vi "ConvertTextBasedCodeToLabVIEW_CreateClasses.vi"(0 "Classes":T11[](array[typedef])=[{"ClassName"="Program", "AccessScope"=enum."public", "Modifiers"=[], "ClassDocumentation"="", "Methods"=[{"ReturnType"={"Name"="", "DataType"=enum."void", "ArrayDim"=0, "CtrlPath"=path "", "DataTypeString"="void", "AccessScope"=enum."public", "InitialData"=variant(string "")}, "MethodName"="Main", "AccessScope"=enum."public", "Modifiers"=[enum."static"], "MethodDocumentation"="", "MethodContent"="public static void Main(string[] args)\n        {\n            // Create a subject and the observable, inject the subject into the observable\n            Subject subject = new Subject();\n            SubjectObservable observable = new SubjectObservable(subject);\n\n            //Create two observers\n            SubjectObserver zeus = new SubjectObserver(observable, \"Zeus\");\n            SubjectObserver ares = new SubjectObserver(observable, \"Ares\");\n            \n            // Run a loop and trigger the observer\n            for (int i = 0; i < 5; i++)\n            {\n                Console.WriteLine(\"Counter: \" + subject.Counter);\n                observable.inspectSubject();\n\n            }\n\n            Console.ReadLine();\n        }", "MethodArguments"=[{"Name"="args", "DataType"=enum."STRING", "ArrayDim"=1, "CtrlPath"=path "", "DataTypeString"="string[]", "AccessScope"=enum."public", "InitialData"=variant(string "")}], "GetProperty"={"Active"=FALSE, "AccessScope"=enum."public", "Code"=""}, "SetProperty"={"Active"=FALSE, "AccessScope"=enum."public", "Code"=""}}], "ParentClasses"=[], "ClassType"=enum."Class", "Owner"="Test", "OwnerType"=enum."Package/NameSpace", "Generics"=[], "Attributes"=[{"Name"="MyUINT8", "DataType"=enum."UINT8", "ArrayDim"=0, "CtrlPath"=path "", "DataTypeString"="", "AccessScope"=enum."public", "InitialData"=variant}], "Enums"=[{"Name"="MyEnum", "AccessScope"=enum."public", "Modifiers"=[], "Items"=["A1", "A2"], "Documentation"="My Enum Doc"}], "Structs"=[{"Name"="MyStruct", "AccessScope"=enum."public", "Modifiers"=[], "Items"=[{"Name"="MyObject", "DataType"=enum."LabVIEW Class", "ArrayDim"=1, "CtrlPath"=path "", "DataTypeString"="Program", "AccessScope"=enum."public", "InitialData"=variant}, {"Name"="Sträng", "DataType"=enum."STRING", "ArrayDim"=0, "CtrlPath"=path "", "DataTypeString"="", "AccessScope"=enum."public", "InitialData"=variant}], "Documentation"="Struct Doc"}]}, {"ClassName"="Subject", "AccessScope"=enum."public", "Modifiers"=[], "ClassDocumentation"="Class Subject - It has a counter object that increases everytime you inspect it", "Methods"=[{"ReturnType"={"Name"="", "DataType"=enum."INT32", "ArrayDim"=0, "CtrlPath"=path "", "DataTypeString"="int", "AccessScope"=enum."public", "InitialData"=variant(string "")}, "MethodName"="Counter", "AccessScope"=enum."public", "Modifiers"=[], "MethodDocumentation"="", "MethodContent"="public int Counter\n        {\n            get\n            {\n                return ++_counter;\n            }\n        }", "MethodArguments"=[], "GetProperty"={"Active"=TRUE, "AccessScope"=enum."public", "Code"="return ++_counter;"}, "SetProperty"={"Active"=FALSE, "AccessScope"=enum."public", "Code"=""}}], "ParentClasses"=[], "ClassType"=enum."Class", "Owner"="Test", "OwnerType"=enum."Package/NameSpace", "Generics"=[], "Attributes"=[{"Name"="_counter", "DataType"=enum."INT32", "ArrayDim"=0, "CtrlPath"=path "", "DataTypeString"="int", "AccessScope"=enum."private", "InitialData"=variant(string "")}], "Enums"=[], "Structs"=[]}, {"ClassName"="SubjectObservable", "AccessScope"=enum."public", "Modifiers"=[], "ClassDocumentation"="Class Subject Observable - The observable object that observes the subject and notifies the observers", "Methods"=[{"ReturnType"={"Name"="", "DataType"=enum."LabVIEW Object", "ArrayDim"=0, "CtrlPath"=path "", "DataTypeString"="SubjectObservable", "AccessScope"=enum."public", "InitialData"=variant(string "")}, "MethodName"="SubjectObservable", "AccessScope"=enum."public", "Modifiers"=[], "MethodDocumentation"="Accept a subject instance which we shall observe", "MethodContent"="public SubjectObservable(Subject subject)\n        {\n            _subjectObservers = new List<IObserver<Subject>>();\n            _subject = subject;\n\n        }", "MethodArguments"=[{"Name"="subject", "DataType"=enum."LabVIEW Object", "ArrayDim"=0, "CtrlPath"=path "", "DataTypeString"="Subject", "AccessScope"=enum."public", "InitialData"=variant(string "")}], "GetProperty"={"Active"=FALSE, "AccessScope"=enum."public", "Code"=""}, "SetProperty"={"Active"=FALSE, "AccessScope"=enum."public", "Code"=""}}, {"ReturnType"={"Name"="", "DataType"=enum."Other", "ArrayDim"=0, "CtrlPath"=path "", "DataTypeString"="IDisposable", "AccessScope"=enum."public", "InitialData"=variant(string "")}, "MethodName"="Subscribe", "AccessScope"=enum."public", "Modifiers"=[], "MethodDocumentation"="This method allows the observers to attach themselves. It returns a disposer object to the observer\nwhich the observer can utilize to unsubscribe", "MethodContent"="public IDisposable Subscribe(IObserver<Subject> observer)\n        {\n            if (!_subjectObservers.Contains(observer))\n            {\n                _subjectObservers.Add(observer);\n            }\n\n            return new Disposer(_subjectObservers, observer);\n        }", "MethodArguments"=[{"Name"="observer", "DataType"=enum."Other", "ArrayDim"=0, "CtrlPath"=path "", "DataTypeString"="IObserver<Subject>", "AccessScope"=enum."public", "InitialData"=variant(string "")}], "GetProperty"={"Active"=FALSE, "AccessScope"=enum."public", "Code"=""}, "SetProperty"={"Active"=FALSE, "AccessScope"=enum."public", "Code"=""}}, {"ReturnType"={"Name"="", "DataType"=enum."void", "ArrayDim"=0, "CtrlPath"=path "", "DataTypeString"="void", "AccessScope"=enum."public", "InitialData"=variant(string "")}, "MethodName"="inspectSubject", "AccessScope"=enum."public", "Modifiers"=[enum."event"], "MethodDocumentation"="This method is used to inspect the subject over time. Usually used with a timer or an event", "MethodContent"="event\n        public void inspectSubject()\n        {\n            foreach (IObserver<Subject> observer in _subjectObservers)\n            {\n                observer.OnNext(_subject);\n            }\n        }", "MethodArguments"=[], "GetProperty"={"Active"=FALSE, "AccessScope"=enum."public", "Code"=""}, "SetProperty"={"Active"=FALSE, "AccessScope"=enum."public", "Code"=""}}], "ParentClasses"=[{"ClassName"="IObservable", "ClassType"=enum."Undefined"}], "ClassType"=enum."Class", "Owner"="Test", "OwnerType"=enum."Package/NameSpace", "Generics"=["Subject"], "Attributes"=[{"Name"="_subjectObservers", "DataType"=enum."Other", "ArrayDim"=1, "CtrlPath"=path "", "DataTypeString"="IObserver<Subject>", "AccessScope"=enum."private", "InitialData"=variant(string "")}, {"Name"="_subject", "DataType"=enum."LabVIEW Object", "ArrayDim"=0, "CtrlPath"=path "", "DataTypeString"="Subject", "AccessScope"=enum."private", "InitialData"=variant(string "")}], "Enums"=[], "Structs"=[]}, {"ClassName"="SubjectObserver", "AccessScope"=enum."public", "Modifiers"=[], "ClassDocumentation"="Class Subject Observer - The object that attaches itself to a observable and recieves notifications", "Methods"=[{"ReturnType"={"Name"="", "DataType"=enum."LabVIEW Object", "ArrayDim"=0, "CtrlPath"=path "", "DataTypeString"="SubjectObserver", "AccessScope"=enum."public", "InitialData"=variant(string "")}, "MethodName"="SubjectObserver", "AccessScope"=enum."public", "Modifiers"=[], "MethodDocumentation"="", "MethodContent"="public SubjectObserver(IObservable<Subject> provider, string instanceName)\n        {\n            if (provider != null)\n            {\n                _disposer = provider.Subscribe(this);\n                _instaceName = instanceName;\n            }\n        }", "MethodArguments"=[{"Name"="provider", "DataType"=enum."Other", "ArrayDim"=0, "CtrlPath"=path "", "DataTypeString"="IObservable<Subject>", "AccessScope"=enum."public", "InitialData"=variant(string "")}, {"Name"="instanceName", "DataType"=enum."STRING", "ArrayDim"=0, "CtrlPath"=path "", "DataTypeString"="string", "AccessScope"=enum."public", "InitialData"=variant(string "")}], "GetProperty"={"Active"=FALSE, "AccessScope"=enum."public", "Code"=""}, "SetProperty"={"Active"=FALSE, "AccessScope"=enum."public", "Code"=""}}, {"ReturnType"={"Name"="", "DataType"=enum."void", "ArrayDim"=0, "CtrlPath"=path "", "DataTypeString"="void", "AccessScope"=enum."public", "InitialData"=variant(string "")}, "MethodName"="OnNext", "AccessScope"=enum."public", "Modifiers"=[], "MethodDocumentation"="The observable invokes this method to pass the Subject object to the observer", "MethodContent"="public void OnNext(Subject value)\n        {\n            Console.WriteLine(\"[\" + _instaceName + \"] \" + value.Counter);\n        }", "MethodArguments"=[{"Name"="value", "DataType"=enum."LabVIEW Object", "ArrayDim"=0, "CtrlPath"=path "", "DataTypeString"="Subject", "AccessScope"=enum."public", "InitialData"=variant(string "")}], "GetProperty"={"Active"=FALSE, "AccessScope"=enum."public", "Code"=""}, "SetProperty"={"Active"=FALSE, "AccessScope"=enum."public", "Code"=""}}, {"ReturnType"={"Name"="", "DataType"=enum."void", "ArrayDim"=0, "CtrlPath"=path "", "DataTypeString"="void", "AccessScope"=enum."public", "InitialData"=variant(string "")}, "MethodName"="OnCompleted", "AccessScope"=enum."public", "Modifiers"=[], "MethodDocumentation"="Usually called when a transmission is complete. Not implemented.", "MethodContent"="public void OnCompleted()\n        {\n            throw new NotImplementedException();\n        }", "MethodArguments"=[], "GetProperty"={"Active"=FALSE, "AccessScope"=enum."public", "Code"=""}, "SetProperty"={"Active"=FALSE, "AccessScope"=enum."public", "Code"=""}}, {"ReturnType"={"Name"="", "DataType"=enum."void", "ArrayDim"=0, "CtrlPath"=path "", "DataTypeString"="void", "AccessScope"=enum."public", "InitialData"=variant(string "")}, "MethodName"="OnError", "AccessScope"=enum."public", "Modifiers"=[], "MethodDocumentation"="Usually called when there was an error. Didn't implement.", "MethodContent"="public void OnError(Exception error)\n        {\n            throw new NotImplementedException();\n        }", "MethodArguments"=[{"Name"="error", "DataType"=enum."Other", "ArrayDim"=0, "CtrlPath"=path "", "DataTypeString"="Exception", "AccessScope"=enum."public", "InitialData"=variant(string "")}], "GetProperty"={"Active"=FALSE, "AccessScope"=enum."public", "Code"=""}, "SetProperty"={"Active"=FALSE, "AccessScope"=enum."public", "Code"=""}}, {"ReturnType"={"Name"="", "DataType"=enum."void", "ArrayDim"=0, "CtrlPath"=path "", "DataTypeString"="void", "AccessScope"=enum."public", "InitialData"=variant(string "")}, "MethodName"="Dispose", "AccessScope"=enum."public", "Modifiers"=[], "MethodDocumentation"="Invoke the disposer recieved from the observable. This will unsubscribe", "MethodContent"="public void Dispose()\n        {\n            _disposer.Dispose();\n        }", "MethodArguments"=[], "GetProperty"={"Active"=FALSE, "AccessScope"=enum."public", "Code"=""}, "SetProperty"={"Active"=FALSE, "AccessScope"=enum."public", "Code"=""}}], "ParentClasses"=[{"ClassName"="IObserver", "ClassType"=enum."Undefined"}], "ClassType"=enum."Class", "Owner"="Test", "OwnerType"=enum."Package/NameSpace", "Generics"=["Subject"], "Attributes"=[{"Name"="_disposer", "DataType"=enum."Other", "ArrayDim"=0, "CtrlPath"=path "", "DataTypeString"="IDisposable", "AccessScope"=enum."private", "InitialData"=variant(string "")}, {"Name"="_instaceName", "DataType"=enum."STRING", "ArrayDim"=0, "CtrlPath"=path "", "DataTypeString"="string", "AccessScope"=enum."private", "InitialData"=variant(string "")}], "Enums"=[], "Structs"=[]}, {"ClassName"="Disposer", "AccessScope"=enum."private", "Modifiers"=[], "ClassDocumentation"="Private class Disposer: Implements the IDisposable. Observable returns an instance to the observer for easy unsubscription\nprivate", "Methods"=[{"ReturnType"={"Name"="", "DataType"=enum."LabVIEW Object", "ArrayDim"=0, "CtrlPath"=path "", "DataTypeString"="Disposer", "AccessScope"=enum."public", "InitialData"=variant(string "")}, "MethodName"="Disposer", "AccessScope"=enum."public", "Modifiers"=[], "MethodDocumentation"="", "MethodContent"="public Disposer(List<IObserver<Subject>> _subObservers, IObserver<Subject> observer)\n            {\n                _subjectObservers = _subObservers;\n                _observer = observer;\n            }", "MethodArguments"=[{"Name"="_subObservers", "DataType"=enum."Other", "ArrayDim"=1, "CtrlPath"=path "", "DataTypeString"="IObserver<Subject>", "AccessScope"=enum."public", "InitialData"=variant(string "")}, {"Name"="observer", "DataType"=enum."Other", "ArrayDim"=0, "CtrlPath"=path "", "DataTypeString"="IObserver<Subject>", "AccessScope"=enum."public", "InitialData"=variant(string "")}], "GetProperty"={"Active"=FALSE, "AccessScope"=enum."public", "Code"=""}, "SetProperty"={"Active"=FALSE, "AccessScope"=enum."public", "Code"=""}}, {"ReturnType"={"Name"="", "DataType"=enum."void", "ArrayDim"=0, "CtrlPath"=path "", "DataTypeString"="void", "AccessScope"=enum."public", "InitialData"=variant(string "")}, "MethodName"="Dispose", "AccessScope"=enum."public", "Modifiers"=[], "MethodDocumentation"="", "MethodContent"="public void Dispose()\n            {\n                if (_subjectObservers.Contains(_observer))\n                {\n                    _subjectObservers.Remove(_observer);\n                }\n            }", "MethodArguments"=[], "GetProperty"={"Active"=FALSE, "AccessScope"=enum."public", "Code"=""}, "SetProperty"={"Active"=FALSE, "AccessScope"=enum."public", "Code"=""}}], "ParentClasses"=[{"ClassName"="IDisposable", "ClassType"=enum."Undefined"}], "ClassType"=enum."Class", "Owner"="SubjectObservable", "OwnerType"=enum."Class", "Generics"=[], "Attributes"=[{"Name"="_subjectObservers", "DataType"=enum."Other", "ArrayDim"=1, "CtrlPath"=path "", "DataTypeString"="IObserver<Subject>", "AccessScope"=enum."private", "InitialData"=variant(string "")}, {"Name"="_observer", "DataType"=enum."Other", "ArrayDim"=0, "CtrlPath"=path "", "DataTypeString"="IObserver<Subject>", "AccessScope"=enum."private", "InitialData"=variant(string "")}], "Enums"=[], "Structs"=[]}], 1 "TopFolder":path=path "D:/Temp", 2 "InterfacesThatShouldBeConvertedToClasses":string[](array[string]), 3 "Options":T7={"ClassProvider"=enum."LabVIEW Native(By value)", "PropertyMethodType"=enum."PropertyMethod", "Pattern type"=2} {"Pattern type" items=["4x4x4", "5x6x5", "6x8x6"]}, 5 "MissingItems":T17[](array[typedef])=[{"Item"="IObservable", "Options"=["Select action to handle missing type", "Create stub code as class", "Create stub code as interface by VI Server", "Remove dependency to this type"], "Icons"=[enum."?", enum."Add", enum."Add", enum."Delete"], "Index"=2}, {"Item"="IDisposable", "Options"=["Select action to handle missing type", "Create stub code as class", "Create stub code as interface by VI Server", "Remove dependency to this type"], "Icons"=[enum."?", enum."Add", enum."Add", enum."Delete"], "Index"=1}, {"Item"="IObserver", "Options"=["Select action to handle missing type", "Create stub code as class", "Create stub code as interface by VI Server", "Remove dependency to this type"], "Icons"=[enum."?", enum."Add", enum."Add", enum."Delete"], "Index"=2}, {"Item"="Exception", "Options"=["Select action to handle missing type", "Create stub code as class", "Remove dependency to this type"], "Icons"=[enum."?", enum."Add", enum."Delete"], "Index"=2}], 7 "BetterNames":bool, 9 "ExistingClassFolders":path[](array[path]), 11 "error in (no error)":errorcluster, 12 "ProgressTextRef":refnum<vi>, 13 "StructsOusideClass":T1[](array[typedef]), 14 "EnumsOusideClass":T6[](array[typedef])) -> (15 "error out":errorcluster)   [LabVIEW 2020]
uses:
  ConvertTextBasedCodeToLabVIEW_MissingType.ctl
  ConvertTextBasedCodeToLabVIEW_MissingTypeIconType.ctl
  String/GDSString_ClassDescriptionType.ctl
  String/GDSString_AccessScopeModifierType.ctl
  String/GDSString_ModifierType.ctl
  String/GDSString_MethodDescriptionType.ctl
  CommonVIs/CommonVIs_AttributeType.ctl
  CommonVIs/CommonVIs_AttributeDataType.ctl
  CommonVIs/CommonVIs_PropertyType.ctl
  String/GDSString_ClassParentType.ctl
  String/GDSString_ClassType.ctl
  String/GDSString_ClassOwnerType.ctl
  CommonVIs/CommonVIs_EnumType.ctl
  CommonVIs/CommonVIs_StructType.ctl
  ConvertTextBasedCodeToLabVIEW_CreateClassesOption.ctl
  API/GDSAPI_SubVIs/GDSAPI_ClassProviderType.ctl
  API/GDSAPI_SubVIs/GDSAPI_PropertyMethodType.ctl
  ScriptingFunctions/Scripting_ConnectorPanePatternType.ctl
  CommonVIs/CommonVIs_ClassNamePathType.ctl
  API/GDSAPI_SubVIs/GDSAPI_SetClassOptionsAction.ctl
  ConvertTextBasedCodeToLabVIEW_MissingTypeOptions.ctl
  API/GDSAPI_CreateInterfaceType.ctl
  Provider_BaseClassInterface/ClassWriter_class/InterfaceMethodsToCreate.ctl
  API/GDSAPI_CreateClassType.ctl
  API/GDSAPI_SubVIs/GDSAPI_ClassTemplateType.ctl
  API/GDSAPI_SubVIs/GDSAPI_ProjectIconType.ctl
  Provider_BaseClassInterface/ClassWriter_class/ClassWriter.lvclass
  <vilib>/zip/NI_Unzip.lvlib
panel:
  out "ClassesOut":T11[](array[typedef])=[{"ClassName"="Program", "AccessScope"=enum."public", "Modifiers"=[], "ClassDocumentation"="", "Methods"=[{"ReturnType"={"Name"="", "DataType"=enum."void", "ArrayDim"=0, "CtrlPath"=path "", "DataTypeString"="void", "AccessScope"=enum."public", "InitialData"=variant(string "")}, "MethodName"="Main", "AccessScope"=enum."public", "Modifiers"=[enum."static"], "MethodDocumentation"="", "MethodContent"="public static void Main(string[] args)\n        {\n            // Create a subject and the observable, inject the subject into the observable\n            Subject subject = new Subject();\n            SubjectObservable observable = new SubjectObservable(subject);\n\n            //Create two observers\n            SubjectObserver zeus = new SubjectObserver(observable, \"Zeus\");\n            SubjectObserver ares = new SubjectObserver(observable, \"Ares\");\n            \n            // Run a loop and trigger the observer\n            for (int i = 0; i < 5; i++)\n            {\n                Console.WriteLine(\"Counter: \" + subject.Counter);\n                observable.inspectSubject();\n\n            }\n\n            Console.ReadLine();\n        }", "MethodArguments"=[{"Name"="args", "DataType"=enum."STRING", "ArrayDim"=1, "CtrlPath"=path "", "DataTypeString"="string[]", "AccessScope"=enum."public", "InitialData"=variant(string "")}], "GetProperty"={"Active"=FALSE, "AccessScope"=enum."public", "Code"=""}, "SetProperty"={"Active"=FALSE, "AccessScope"=enum."public", "Code"=""}}], "ParentClasses"=[], "ClassType"=enum."Class", "Owner"="Test", "OwnerType"=enum."Package/NameSpace", "Generics"=[], "Attributes"=[{"Name"="MyUINT8", "DataType"=enum."UINT8", "ArrayDim"=0, "CtrlPath"=path "", "DataTypeString"="", "AccessScope"=enum."public", "InitialData"=variant}], "Enums"=[{"Name"="MyEnum", "AccessScope"=enum."public", "Modifiers"=[], "Items"=["A1", "A2"], "Documentation"="My Enum Doc"}], "Structs"=[{"Name"="MyStruct", "AccessScope"=enum."public", "Modifiers"=[], "Items"=[{"Name"="MyObject", "DataType"=enum."LabVIEW Class", "ArrayDim"=1, "CtrlPath"=path "", "DataTypeString"="Program", "AccessScope"=enum."public", "InitialData"=variant}, {"Name"="Sträng", "DataType"=enum."STRING", "ArrayDim"=0, "CtrlPath"=path "", "DataTypeString"="", "AccessScope"=enum."public", "InitialData"=variant}], "Documentation"="Struct Doc"}]}, {"ClassName"="Subject", "AccessScope"=enum."public", "Modifiers"=[], "ClassDocumentation"="Class Subject - It has a counter object that increases everytime you inspect it", "Methods"=[{"ReturnType"={"Name"="", "DataType"=enum."INT32", "ArrayDim"=0, "CtrlPath"=path "", "DataTypeString"="int", "AccessScope"=enum."public", "InitialData"=variant(string "")}, "MethodName"="Counter", "AccessScope"=enum."public", "Modifiers"=[], "MethodDocumentation"="", "MethodContent"="public int Counter\n        {\n            get\n            {\n                return ++_counter;\n            }\n        }", "MethodArguments"=[], "GetProperty"={"Active"=TRUE, "AccessScope"=enum."public", "Code"="return ++_counter;"}, "SetProperty"={"Active"=FALSE, "AccessScope"=enum."public", "Code"=""}}], "ParentClasses"=[], "ClassType"=enum."Class", "Owner"="Test", "OwnerType"=enum."Package/NameSpace", "Generics"=[], "Attributes"=[{"Name"="_counter", "DataType"=enum."INT32", "ArrayDim"=0, "CtrlPath"=path "", "DataTypeString"="int", "AccessScope"=enum."private", "InitialData"=variant(string "")}], "Enums"=[], "Structs"=[]}, {"ClassName"="SubjectObservable", "AccessScope"=enum."public", "Modifiers"=[], "ClassDocumentation"="Class Subject Observable - The observable object that observes the subject and notifies the observers", "Methods"=[{"ReturnType"={"Name"="", "DataType"=enum."LabVIEW Object", "ArrayDim"=0, "CtrlPath"=path "", "DataTypeString"="SubjectObservable", "AccessScope"=enum."public", "InitialData"=variant(string "")}, "MethodName"="SubjectObservable", "AccessScope"=enum."public", "Modifiers"=[], "MethodDocumentation"="Accept a subject instance which we shall observe", "MethodContent"="public SubjectObservable(Subject subject)\n        {\n            _subjectObservers = new List<IObserver<Subject>>();\n            _subject = subject;\n\n        }", "MethodArguments"=[{"Name"="subject", "DataType"=enum."LabVIEW Object", "ArrayDim"=0, "CtrlPath"=path "", "DataTypeString"="Subject", "AccessScope"=enum."public", "InitialData"=variant(string "")}], "GetProperty"={"Active"=FALSE, "AccessScope"=enum."public", "Code"=""}, "SetProperty"={"Active"=FALSE, "AccessScope"=enum."public", "Code"=""}}, {"ReturnType"={"Name"="", "DataType"=enum."Other", "ArrayDim"=0, "CtrlPath"=path "", "DataTypeString"="IDisposable", "AccessScope"=enum."public", "InitialData"=variant(string "")}, "MethodName"="Subscribe", "AccessScope"=enum."public", "Modifiers"=[], "MethodDocumentation"="This method allows the observers to attach themselves. It returns a disposer object to the observer\nwhich the observer can utilize to unsubscribe", "MethodContent"="public IDisposable Subscribe(IObserver<Subject> observer)\n        {\n            if (!_subjectObservers.Contains(observer))\n            {\n                _subjectObservers.Add(observer);\n            }\n\n            return new Disposer(_subjectObservers, observer);\n        }", "MethodArguments"=[{"Name"="observer", "DataType"=enum."Other", "ArrayDim"=0, "CtrlPath"=path "", "DataTypeString"="IObserver<Subject>", "AccessScope"=enum."public", "InitialData"=variant(string "")}], "GetProperty"={"Active"=FALSE, "AccessScope"=enum."public", "Code"=""}, "SetProperty"={"Active"=FALSE, "AccessScope"=enum."public", "Code"=""}}, {"ReturnType"={"Name"="", "DataType"=enum."void", "ArrayDim"=0, "CtrlPath"=path "", "DataTypeString"="void", "AccessScope"=enum."public", "InitialData"=variant(string "")}, "MethodName"="inspectSubject", "AccessScope"=enum."public", "Modifiers"=[enum."event"], "MethodDocumentation"="This method is used to inspect the subject over time. Usually used with a timer or an event", "MethodContent"="event\n        public void inspectSubject()\n        {\n            foreach (IObserver<Subject> observer in _subjectObservers)\n            {\n                observer.OnNext(_subject);\n            }\n        }", "MethodArguments"=[], "GetProperty"={"Active"=FALSE, "AccessScope"=enum."public", "Code"=""}, "SetProperty"={"Active"=FALSE, "AccessScope"=enum."public", "Code"=""}}], "ParentClasses"=[{"ClassName"="IObservable", "ClassType"=enum."Undefined"}], "ClassType"=enum."Class", "Owner"="Test", "OwnerType"=enum."Package/NameSpace", "Generics"=["Subject"], "Attributes"=[{"Name"="_subjectObservers", "DataType"=enum."Other", "ArrayDim"=1, "CtrlPath"=path "", "DataTypeString"="IObserver<Subject>", "AccessScope"=enum."private", "InitialData"=variant(string "")}, {"Name"="_subject", "DataType"=enum."LabVIEW Object", "ArrayDim"=0, "CtrlPath"=path "", "DataTypeString"="Subject", "AccessScope"=enum."private", "InitialData"=variant(string "")}], "Enums"=[], "Structs"=[]}, {"ClassName"="SubjectObserver", "AccessScope"=enum."public", "Modifiers"=[], "ClassDocumentation"="Class Subject Observer - The object that attaches itself to a observable and recieves notifications", "Methods"=[{"ReturnType"={"Name"="", "DataType"=enum."LabVIEW Object", "ArrayDim"=0, "CtrlPath"=path "", "DataTypeString"="SubjectObserver", "AccessScope"=enum."public", "InitialData"=variant(string "")}, "MethodName"="SubjectObserver", "AccessScope"=enum."public", "Modifiers"=[], "MethodDocumentation"="", "MethodContent"="public SubjectObserver(IObservable<Subject> provider, string instanceName)\n        {\n            if (provider != null)\n            {\n                _disposer = provider.Subscribe(this);\n                _instaceName = instanceName;\n            }\n        }", "MethodArguments"=[{"Name"="provider", "DataType"=enum."Other", "ArrayDim"=0, "CtrlPath"=path "", "DataTypeString"="IObservable<Subject>", "AccessScope"=enum."public", "InitialData"=variant(string "")}, {"Name"="instanceName", "DataType"=enum."STRING", "ArrayDim"=0, "CtrlPath"=path "", "DataTypeString"="string", "AccessScope"=enum."public", "InitialData"=variant(string "")}], "GetProperty"={"Active"=FALSE, "AccessScope"=enum."public", "Code"=""}, "SetProperty"={"Active"=FALSE, "AccessScope"=enum."public", "Code"=""}}, {"ReturnType"={"Name"="", "DataType"=enum."void", "ArrayDim"=0, "CtrlPath"=path "", "DataTypeString"="void", "AccessScope"=enum."public", "InitialData"=variant(string "")}, "MethodName"="OnNext", "AccessScope"=enum."public", "Modifiers"=[], "MethodDocumentation"="The observable invokes this method to pass the Subject object to the observer", "MethodContent"="public void OnNext(Subject value)\n        {\n            Console.WriteLine(\"[\" + _instaceName + \"] \" + value.Counter);\n        }", "MethodArguments"=[{"Name"="value", "DataType"=enum."LabVIEW Object", "ArrayDim"=0, "CtrlPath"=path "", "DataTypeString"="Subject", "AccessScope"=enum."public", "InitialData"=variant(string "")}], "GetProperty"={"Active"=FALSE, "AccessScope"=enum."public", "Code"=""}, "SetProperty"={"Active"=FALSE, "AccessScope"=enum."public", "Code"=""}}, {"ReturnType"={"Name"="", "DataType"=enum."void", "ArrayDim"=0, "CtrlPath"=path "", "DataTypeString"="void", "AccessScope"=enum."public", "InitialData"=variant(string "")}, "MethodName"="OnCompleted", "AccessScope"=enum."public", "Modifiers"=[], "MethodDocumentation"="Usually called when a transmission is complete. Not implemented.", "MethodContent"="public void OnCompleted()\n        {\n            throw new NotImplementedException();\n        }", "MethodArguments"=[], "GetProperty"={"Active"=FALSE, "AccessScope"=enum."public", "Code"=""}, "SetProperty"={"Active"=FALSE, "AccessScope"=enum."public", "Code"=""}}, {"ReturnType"={"Name"="", "DataType"=enum."void", "ArrayDim"=0, "CtrlPath"=path "", "DataTypeString"="void", "AccessScope"=enum."public", "InitialData"=variant(string "")}, "MethodName"="OnError", "AccessScope"=enum."public", "Modifiers"=[], "MethodDocumentation"="Usually called when there was an error. Didn't implement.", "MethodContent"="public void OnError(Exception error)\n        {\n            throw new NotImplementedException();\n        }", "MethodArguments"=[{"Name"="error", "DataType"=enum."Other", "ArrayDim"=0, "CtrlPath"=path "", "DataTypeString"="Exception", "AccessScope"=enum."public", "InitialData"=variant(string "")}], "GetProperty"={"Active"=FALSE, "AccessScope"=enum."public", "Code"=""}, "SetProperty"={"Active"=FALSE, "AccessScope"=enum."public", "Code"=""}}, {"ReturnType"={"Name"="", "DataType"=enum."void", "ArrayDim"=0, "CtrlPath"=path "", "DataTypeString"="void", "AccessScope"=enum."public", "InitialData"=variant(string "")}, "MethodName"="Dispose", "AccessScope"=enum."public", "Modifiers"=[], "MethodDocumentation"="Invoke the disposer recieved from the observable. This will unsubscribe", "MethodContent"="public void Dispose()\n        {\n            _disposer.Dispose();\n        }", "MethodArguments"=[], "GetProperty"={"Active"=FALSE, "AccessScope"=enum."public", "Code"=""}, "SetProperty"={"Active"=FALSE, "AccessScope"=enum."public", "Code"=""}}], "ParentClasses"=[{"ClassName"="IObserver", "ClassType"=enum."Undefined"}], "ClassType"=enum."Class", "Owner"="Test", "OwnerType"=enum."Package/NameSpace", "Generics"=["Subject"], "Attributes"=[{"Name"="_disposer", "DataType"=enum."Other", "ArrayDim"=0, "CtrlPath"=path "", "DataTypeString"="IDisposable", "AccessScope"=enum."private", "InitialData"=variant(string "")}, {"Name"="_instaceName", "DataType"=enum."STRING", "ArrayDim"=0, "CtrlPath"=path "", "DataTypeString"="string", "AccessScope"=enum."private", "InitialData"=variant(string "")}], "Enums"=[], "Structs"=[]}, {"ClassName"="Disposer", "AccessScope"=enum."private", "Modifiers"=[], "ClassDocumentation"="Private class Disposer: Implements the IDisposable. Observable returns an instance to the observer for easy unsubscription\nprivate", "Methods"=[{"ReturnType"={"Name"="", "DataType"=enum."LabVIEW Object", "ArrayDim"=0, "CtrlPath"=path "", "DataTypeString"="Disposer", "AccessScope"=enum."public", "InitialData"=variant(string "")}, "MethodName"="Disposer", "AccessScope"=enum."public", "Modifiers"=[], "MethodDocumentation"="", "MethodContent"="public Disposer(List<IObserver<Subject>> _subObservers, IObserver<Subject> observer)\n            {\n                _subjectObservers = _subObservers;\n                _observer = observer;\n            }", "MethodArguments"=[{"Name"="_subObservers", "DataType"=enum."Other", "ArrayDim"=1, "CtrlPath"=path "", "DataTypeString"="IObserver<Subject>", "AccessScope"=enum."public", "InitialData"=variant(string "")}, {"Name"="observer", "DataType"=enum."Other", "ArrayDim"=0, "CtrlPath"=path "", "DataTypeString"="IObserver<Subject>", "AccessScope"=enum."public", "InitialData"=variant(string "")}], "GetProperty"={"Active"=FALSE, "AccessScope"=enum."public", "Code"=""}, "SetProperty"={"Active"=FALSE, "AccessScope"=enum."public", "Code"=""}}, {"ReturnType"={"Name"="", "DataType"=enum."void", "ArrayDim"=0, "CtrlPath"=path "", "DataTypeString"="void", "AccessScope"=enum."public", "InitialData"=variant(string "")}, "MethodName"="Dispose", "AccessScope"=enum."public", "Modifiers"=[], "MethodDocumentation"="", "MethodContent"="public void Dispose()\n            {\n                if (_subjectObservers.Contains(_observer))\n                {\n                    _subjectObservers.Remove(_observer);\n                }\n            }", "MethodArguments"=[], "GetProperty"={"Active"=FALSE, "AccessScope"=enum."public", "Code"=""}, "SetProperty"={"Active"=FALSE, "AccessScope"=enum."public", "Code"=""}}], "ParentClasses"=[{"ClassName"="IDisposable", "ClassType"=enum."Undefined"}], "ClassType"=enum."Class", "Owner"="SubjectObservable", "OwnerType"=enum."Class", "Generics"=[], "Attributes"=[{"Name"="_subjectObservers", "DataType"=enum."Other", "ArrayDim"=1, "CtrlPath"=path "", "DataTypeString"="IObserver<Subject>", "AccessScope"=enum."private", "InitialData"=variant(string "")}, {"Name"="_observer", "DataType"=enum."Other", "ArrayDim"=0, "CtrlPath"=path "", "DataTypeString"="IObserver<Subject>", "AccessScope"=enum."private", "InitialData"=variant(string "")}], "Enums"=[], "Structs"=[]}]
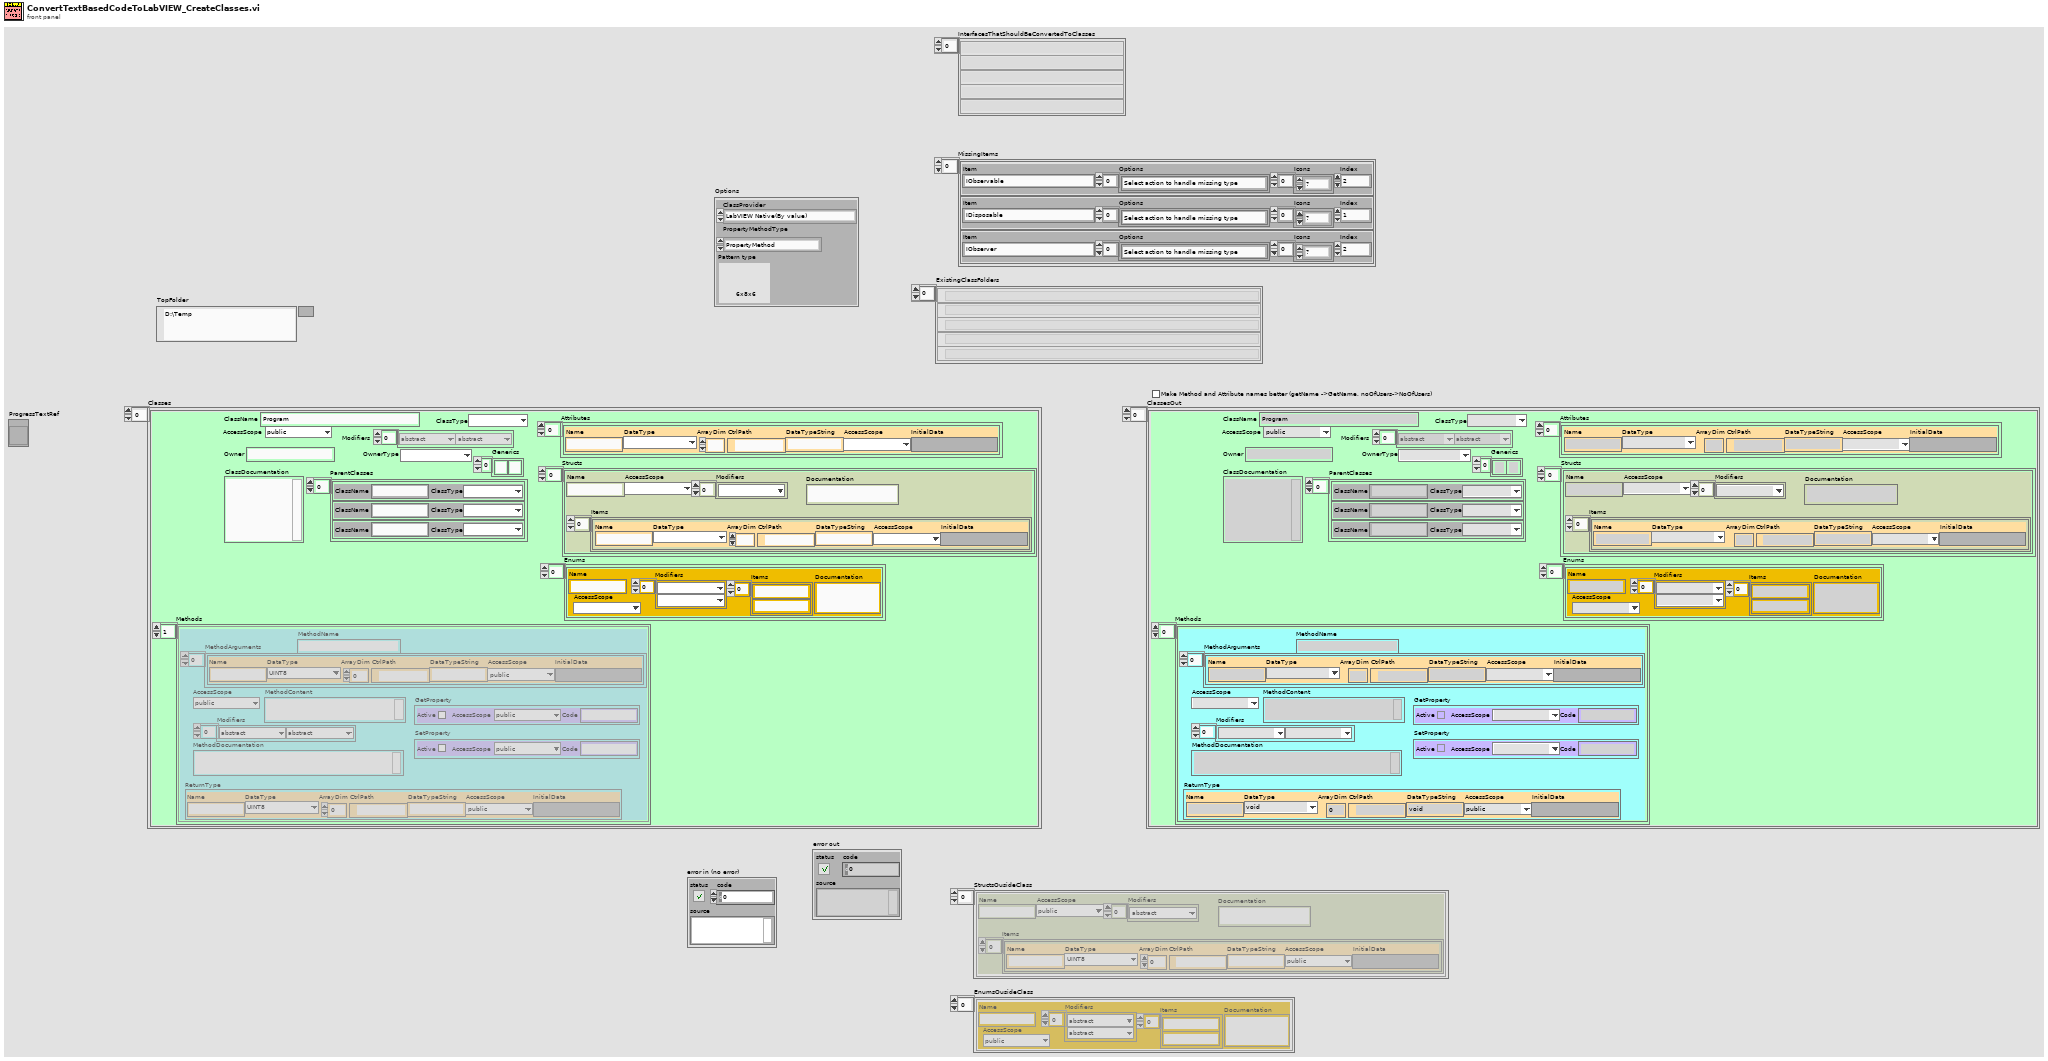
[diagram p1: front panel]
types:
  T1 = typedef "CommonVIs_StructType.ctl" = cluster{"Name":string, "AccessScope":T2, "Modifiers":T3[], "Items":T4[], "Documentation":string}
  T2 = typedef "GDSString_AccessScopeModifierType.ctl" = enum16{"public", "private", "protected", "internal"}
  T3 = typedef "GDSString_ModifierType.ctl" = enum16{"abstract", "static", "final", "synchronized", "strictfp", "async", "const", "event", "extern", "new", "native ", "override", "partial", "readonly", "sealed", "unsafe", "virtual", "volatile"}
  T4 = typedef "CommonVIs_AttributeType.ctl" = cluster{"Name":string, "DataType":T5, "ArrayDim":i32, "CtrlPath":path, "DataTypeString":string, "AccessScope":T2, "InitialData":variant}
  T5 = typedef "CommonVIs_AttributeDataType.ctl" = enum16{"UINT8", "INT8", "UINT16", "INT16", "UINT32", "INT32", "UINT64", "INT64", "SGL", "DBL", "EXT", "CSG", "CDB", "CXT", "TimeStamp", "STRING", "PATH", "BOOL", "ENUM", "RefNum", "VIRefNum", "LabVIEW Class", "Cluster", "Variant", "TypeDef", "Waveform", "LabVIEW Object", "Other", "void", "Set", "Map"}
  T6 = typedef "CommonVIs_EnumType.ctl" = cluster{"Name":string, "AccessScope":T2, "Modifiers":T3[], "Items":string[], "Documentation":string}
  T7 = typedef "ConvertTextBasedCodeToLabVIEW_CreateClassesOption.ctl" = cluster{"ClassProvider":T8, "PropertyMethodType":T9, "Pattern type":T10}
  T8 = typedef "GDSAPI_ClassProviderType.ctl" = enum16{"LabVIEW Native(By value)", "GOOP-3(By reference)", "GOOP-4(By reference)"}
  T9 = typedef "GDSAPI_PropertyMethodType.ctl" = enum16{"PropertyMethod", "PropertyNode"}
  T10 = typedef "Scripting_ConnectorPanePatternType.ctl" = u16
  T11 = typedef "GDSString_ClassDescriptionType.ctl" = cluster{"ClassName":string, "AccessScope":T2, "Modifiers":T3[], "ClassDocumentation":string, "Methods":T12[], "ParentClasses":T14[], "ClassType":T15, "Owner":string, "OwnerType":T16, "Generics":string[], "Attributes":T4[], "Enums":T6[], "Structs":T1[]}
  T12 = typedef "GDSString_MethodDescriptionType.ctl" = cluster{"ReturnType":T4, "MethodName":string, "AccessScope":T2, "Modifiers":T3[], "MethodDocumentation":string, "MethodContent":string, "MethodArguments":T4[], "GetProperty":T13, "SetProperty":T13}
  T13 = typedef "CommonVIs_PropertyType.ctl" = cluster{"Active":bool, "AccessScope":T2, "Code":string}
  T14 = typedef "GDSString_ClassParentType.ctl" = cluster{"ClassName":string, "ClassType":T15}
  T15 = typedef "GDSString_ClassType.ctl" = enum16{"Undefined", "Class", "Interface"}
  T16 = typedef "GDSString_ClassOwnerType.ctl" = enum16{"NoOwner", "Class", "Package/NameSpace"}
  T17 = typedef "ConvertTextBasedCodeToLabVIEW_MissingType.ctl" = cluster{"Item":string, "Options":string[], "Icons":T18[], "Index":i32}
  T18 = typedef "ConvertTextBasedCodeToLabVIEW_MissingTypeIconType.ctl" = enum16{"?", "Add", "Delete", "Implement", "Inherit"}
  T19 = typedef "GDSAPI_SetClassOptionsAction.ctl" = enum16{"Set All", "Set Project Icon Type", "Set Pattern Type", "Set Wire Configuration"}
  T20 = typedef "CommonVIs_ClassNamePathType.ctl" = cluster{"ClassNamn":string, "ClassPath":path, "InterfaceClass":bool}
  T21 = cluster{"App":refnum<vi>, "Proj":refnum<vi>, "ClassesToCreate":string[], "StructsToCreate":string[], "EnumsToCreate":string[], "Classes":T11[], "ProjItem":refnum<vi>, "ClassPath":path[], "ExistingClasses/Types":string[], "ClassRefs":refnum<vi>[], "ClassInfo":T20[], "StartTime":timestamp, "MissingTypes":string[], "Pattern-Before":T10, "ClassesStart":T11[]}
  T22 = typedef "GDSAPI_ProjectIconType.ctl" = enum16{"BlueCircle", "BlueFrame", "BlueFull", "BlueMessage", "BrownCircle", "BrownFrame", "BrownFull", "BurgundyCircle", "BurgundyFrame", "BurgundyFull", "CyanCircle", "CyanFrame", "CyanFull", "DarkBlueCircle", "DarkBlueFrame", "DarkBlueFull", "ForestGreenCircle", "ForestGreenFrame", "ForestGreenFull", "GrayCircle", "GrayFrame", "GrayFull", "GreenCircle", "GreenFrame", "GreenFull", "Interface", "InterfaceBlue", "InterfaceBrown", "InterfaceBurgundy", "InterfaceCyan", "InterfaceDarkBlue", "InterfaceForestGreen", "InterfaceGray", "InterfaceGreen", "InterfaceLightGreen", "InterfaceLightRed", "InterfacePink", "InterfacePurple", "InterfaceRed", "InterfaceYellow", "LightGreenCircle", "LightGreenFrame", "LightGreenFull", "LightRedCircle", "LightRedFrame", "LightRedFull", "PinkCircle", "PinkFrame", "PinkFull", "PurpleCircle", "PurpleFrame", "PurpleFull", "RedCircle", "RedFrame", "RedFull", "YellowCircle", "YellowFrame", "YellowFull"}
  T23 = typedef "ConvertTextBasedCodeToLabVIEW_MissingTypeOptions.ctl" = enum16{"Select action to handle missing type", "Create stub code as class", "Create stub code as interface", "Remove dependency to this type"}
  T24 = typedef "GDSAPI_CreateInterfaceType.ctl" = cluster{"NewInterfaceFolder":path, "InterfaceName":string, "InterfaceDescription":string, "ParentInterfacesFilePath":path[], "FolderSuffix":string, "MethodsToCreate":T25[]}
  T25 = typedef "ClassWriter.lvclass/InterfaceMethodsToCreate.ctl" = cluster{"Name":string, "Description":string, "MethodsArgumentsIn":T4[], "MethodsArgumentsOut":T4[], "DecendantsMustOverride":bool}
  T26 = typedef "GDSAPI_CreateClassType.ctl" = cluster{"ClassProvider":T8, "NewClassFolder":path, "ParentLvClassFilePath":path, "ClassName":string, "ClassDescription":string, "ClassTemplate":T27, "ParentInterfacesFilePath":path[]}
  T27 = typedef "GDSAPI_ClassTemplateType.ctl" = enum16{"Standard", "Singleton"}
  T28 = cluster{"ClassName":string, "SearchPattern":string[]}[]
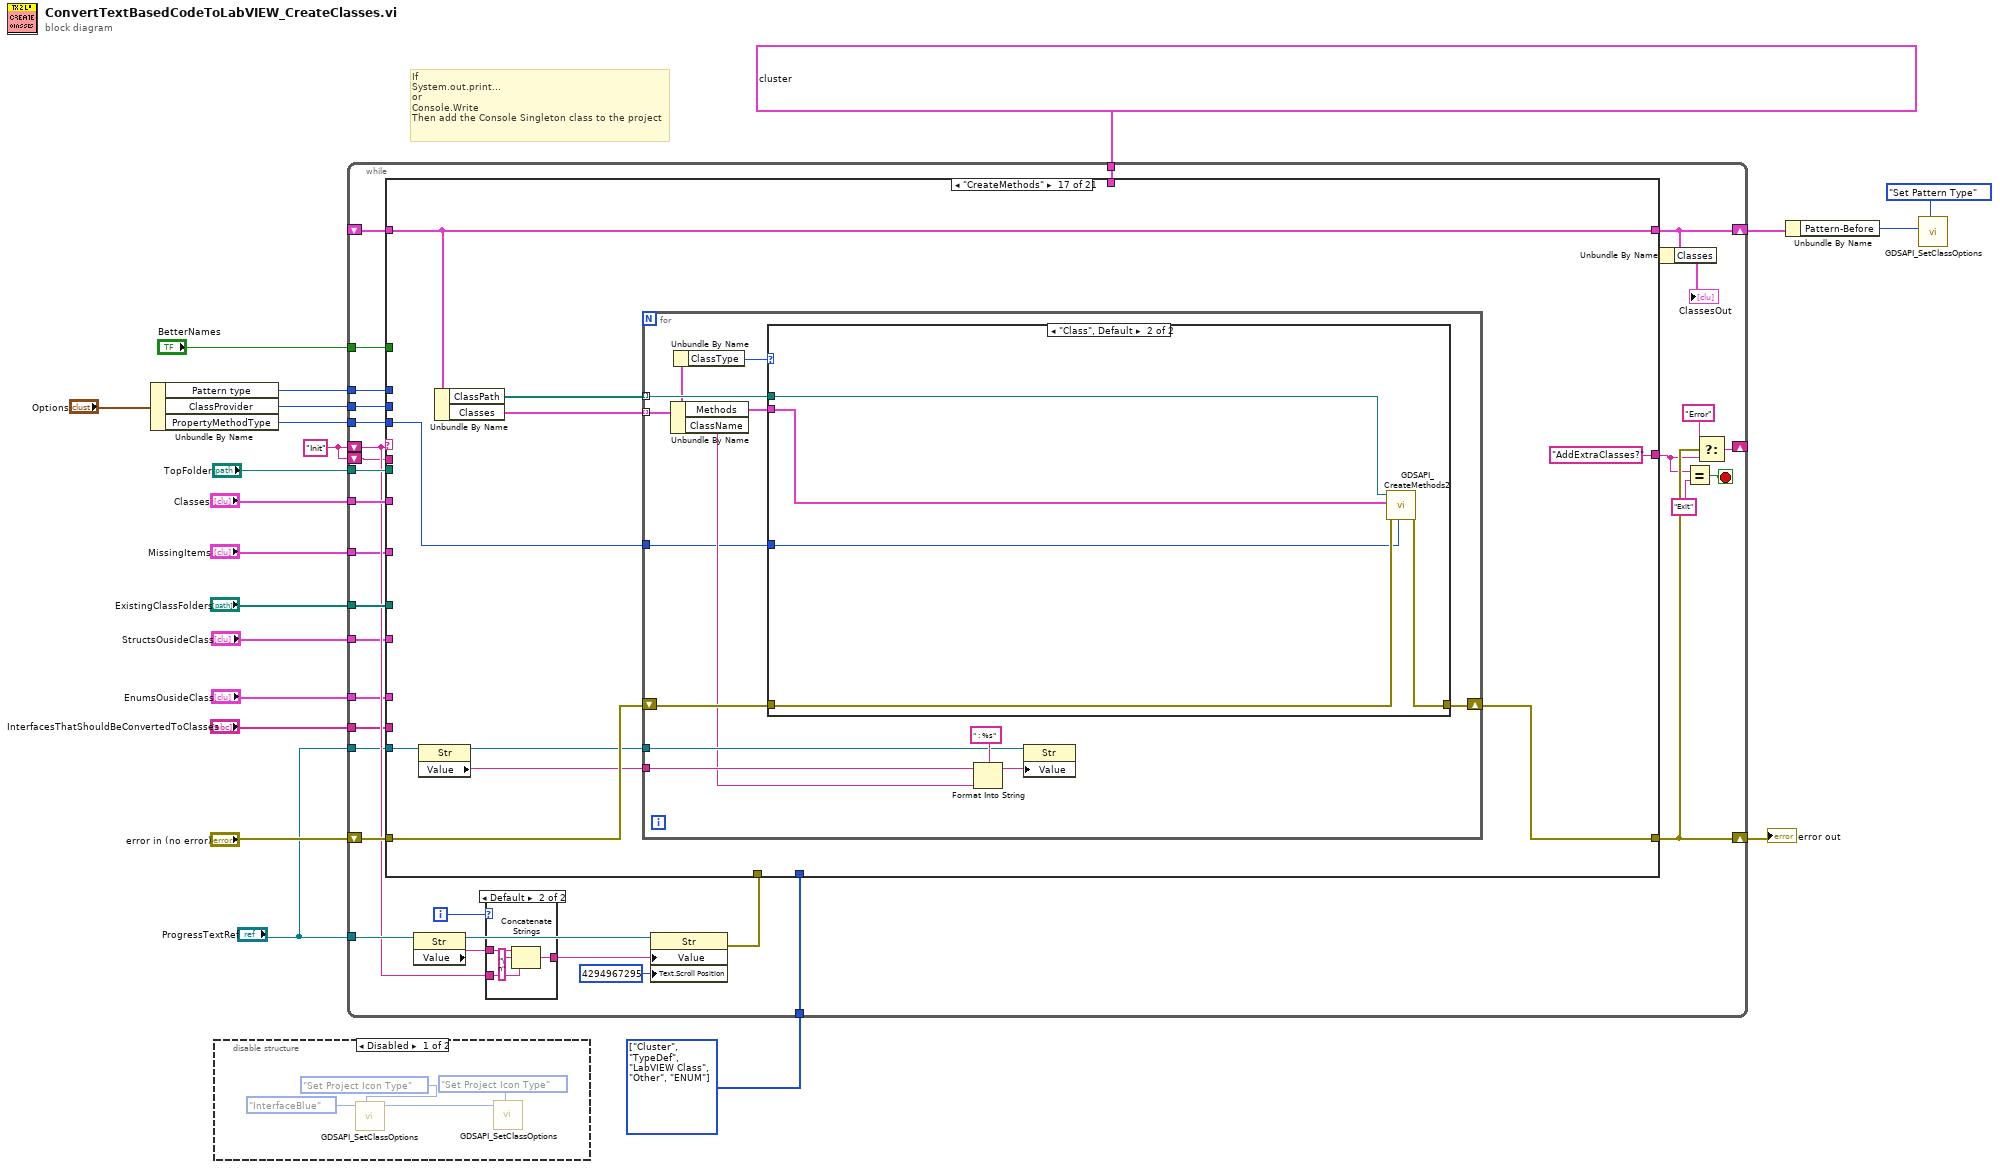
[diagram p0: block diagram]
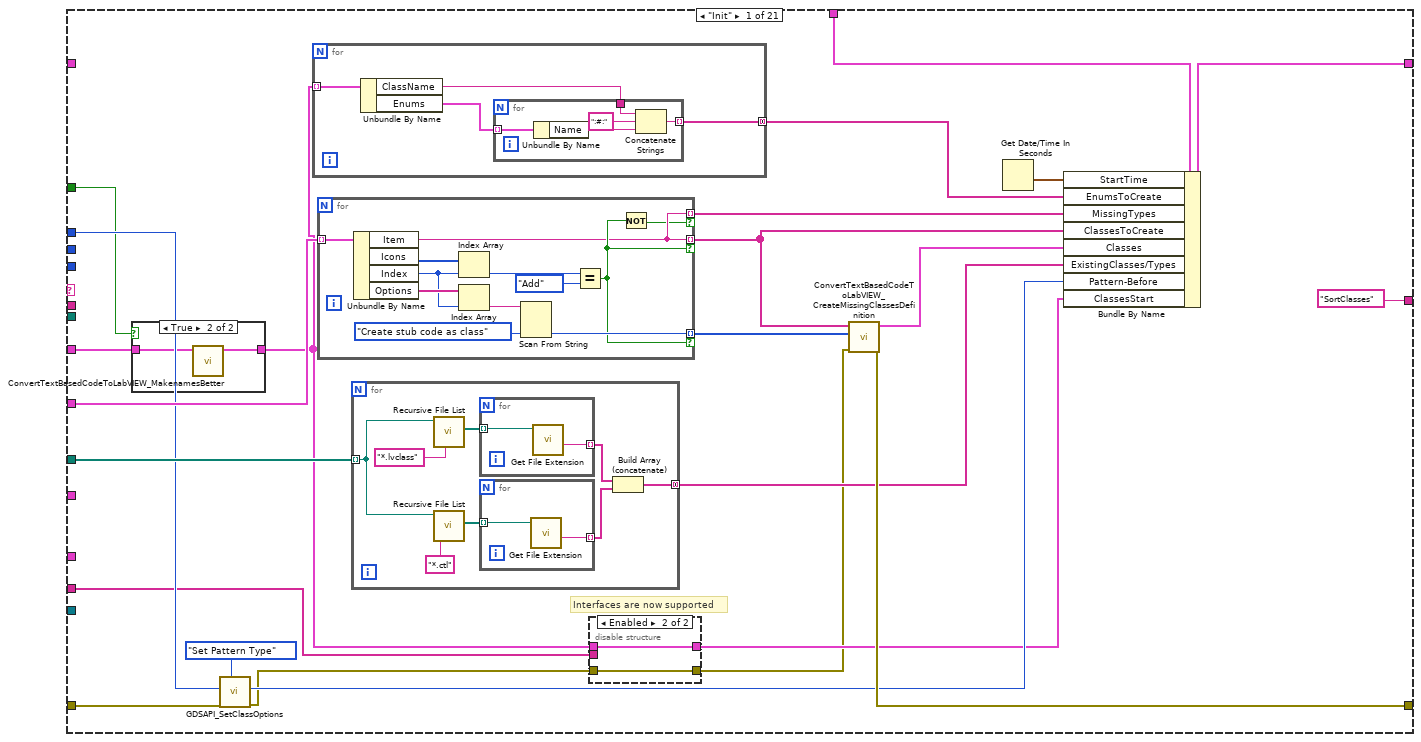
[diagram p4: hidden frame]
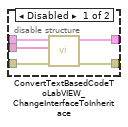
[diagram p5: hidden frame]
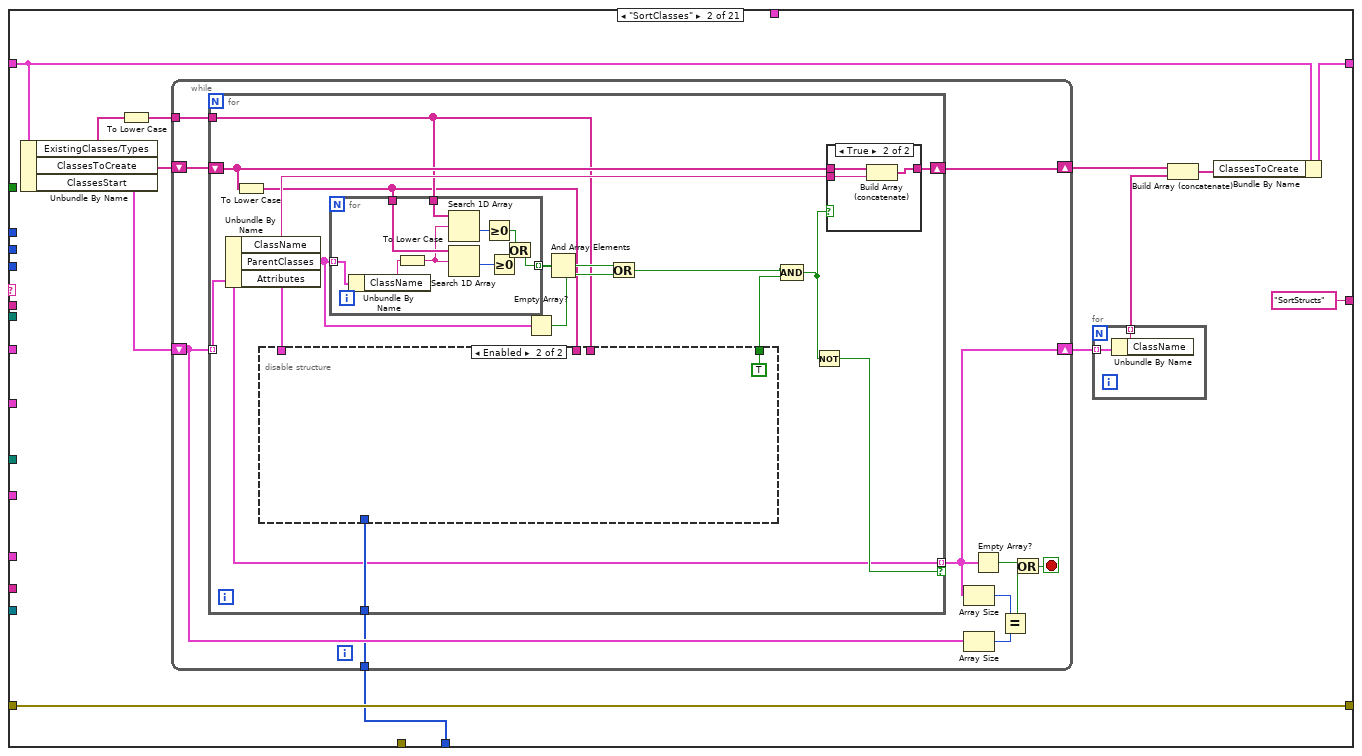
[diagram p7: hidden frame]
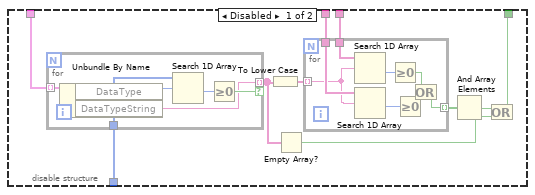
[diagram p8: hidden frame]
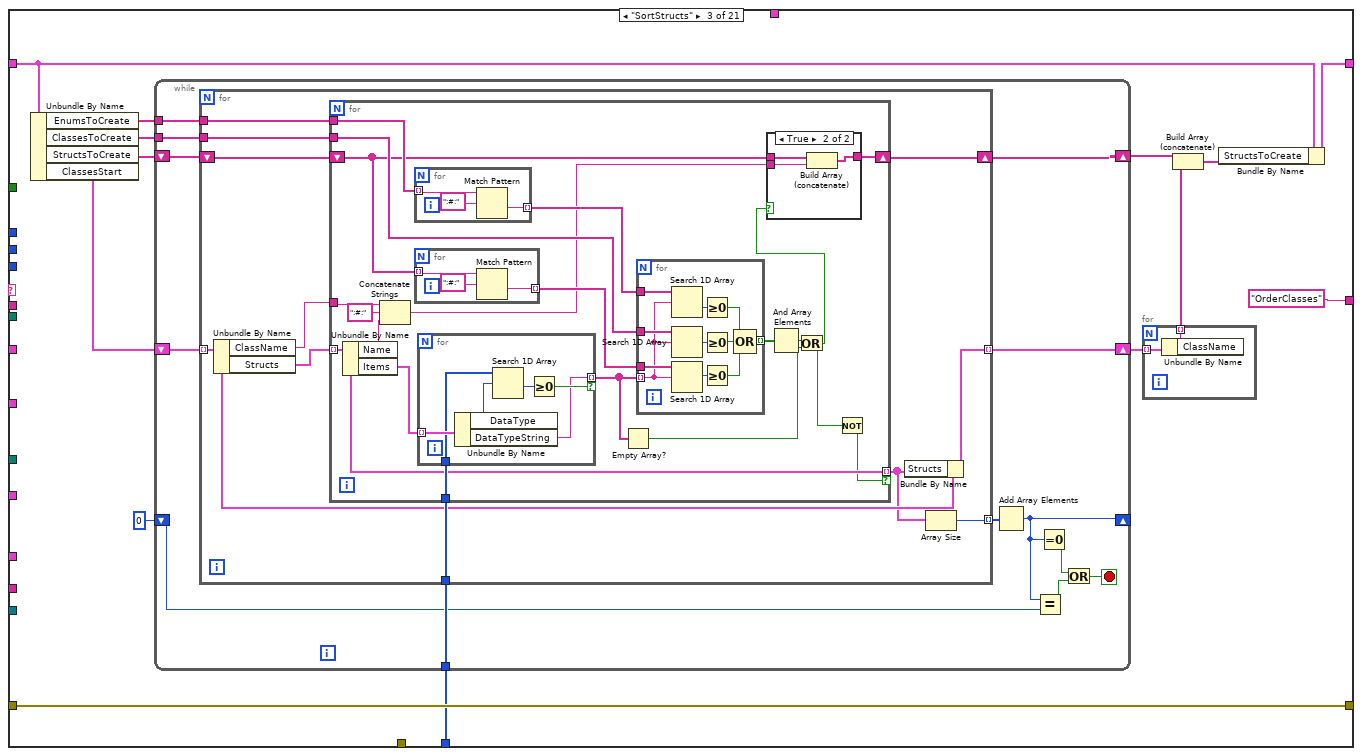
[diagram p10: hidden frame]
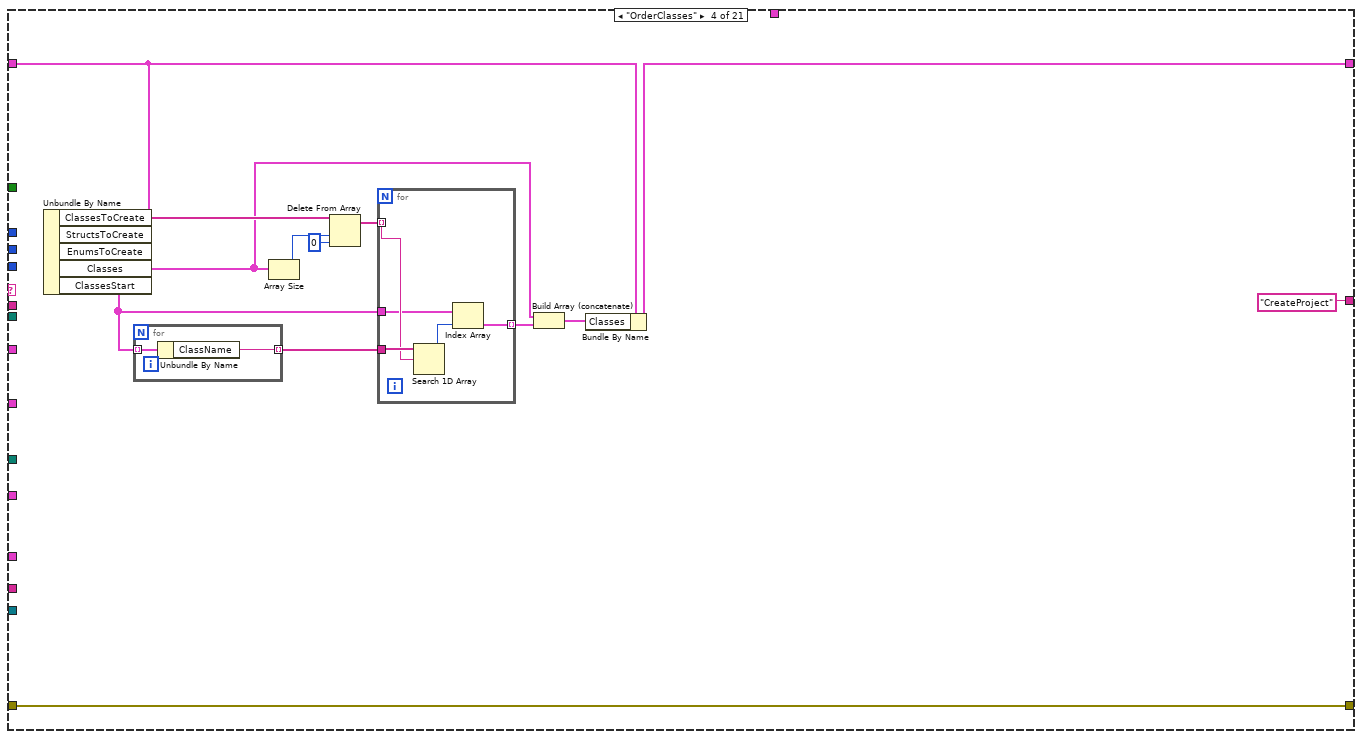
[diagram p12: hidden frame]
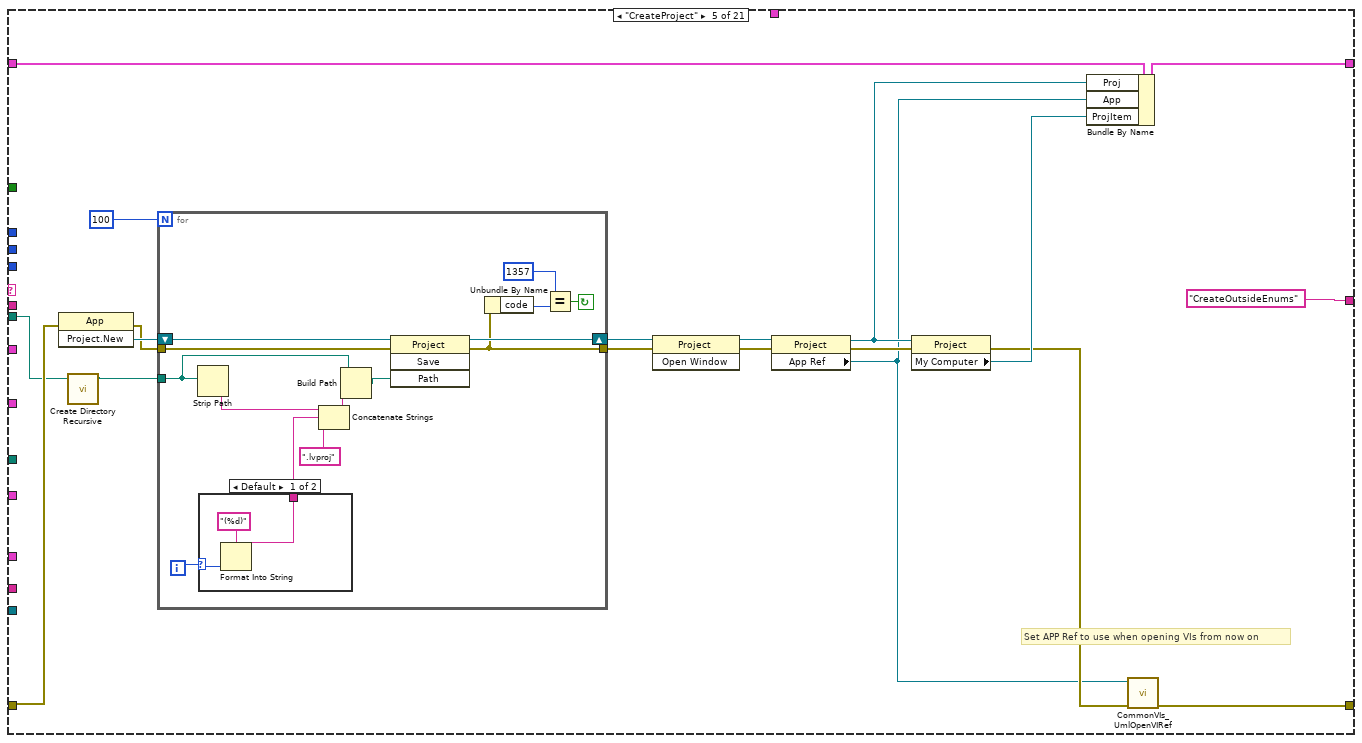
[diagram p13: hidden frame]
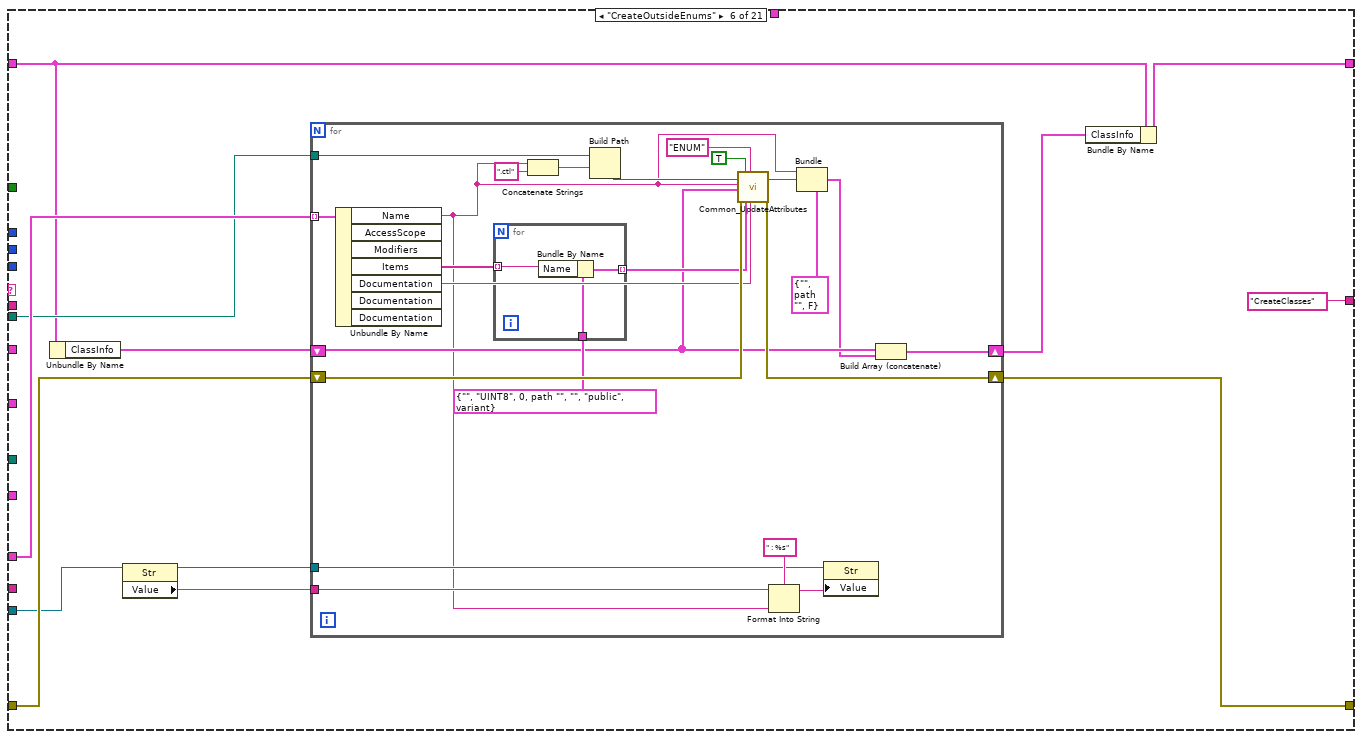
[diagram p15: hidden frame]
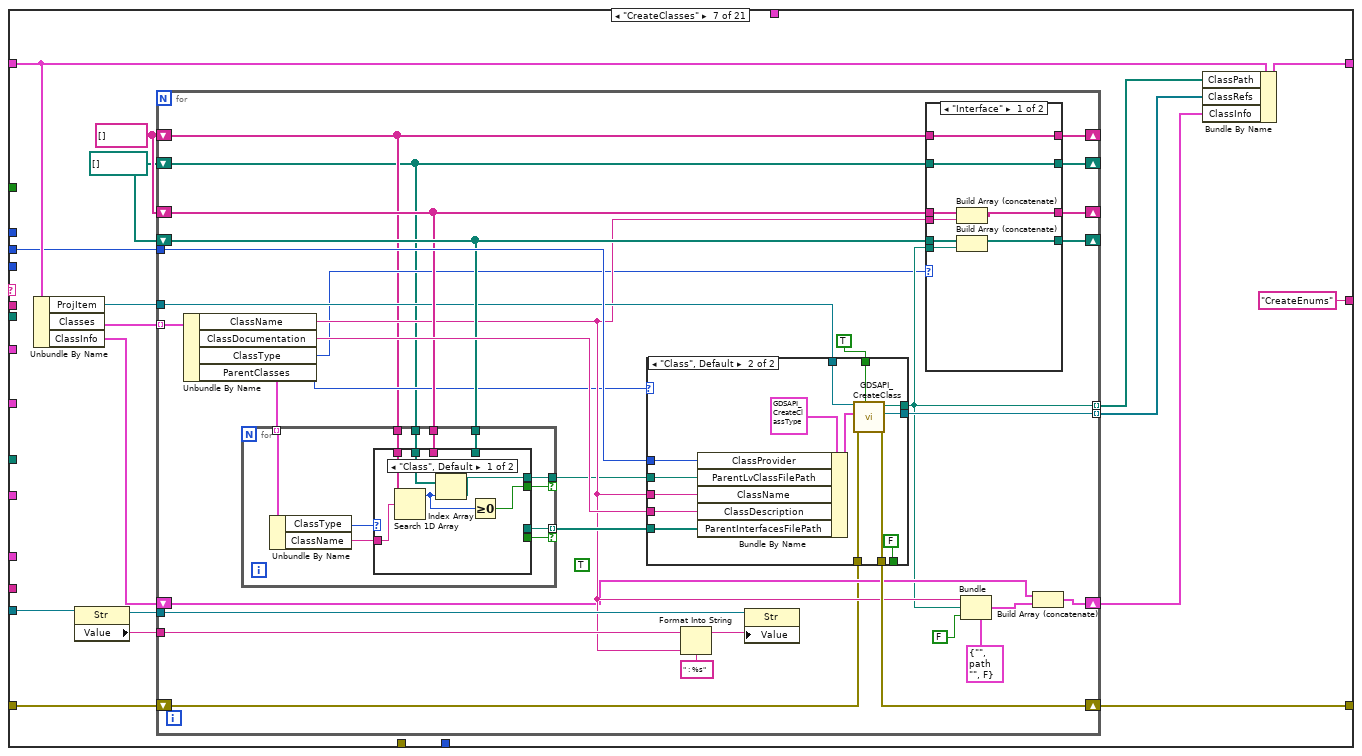
[diagram p16: hidden frame]
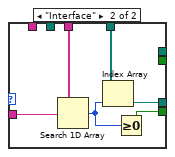
[diagram p17: hidden frame]
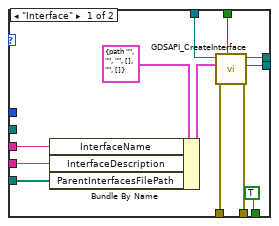
[diagram p18: hidden frame]
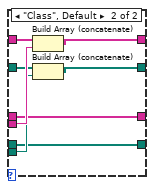
[diagram p19: hidden frame]
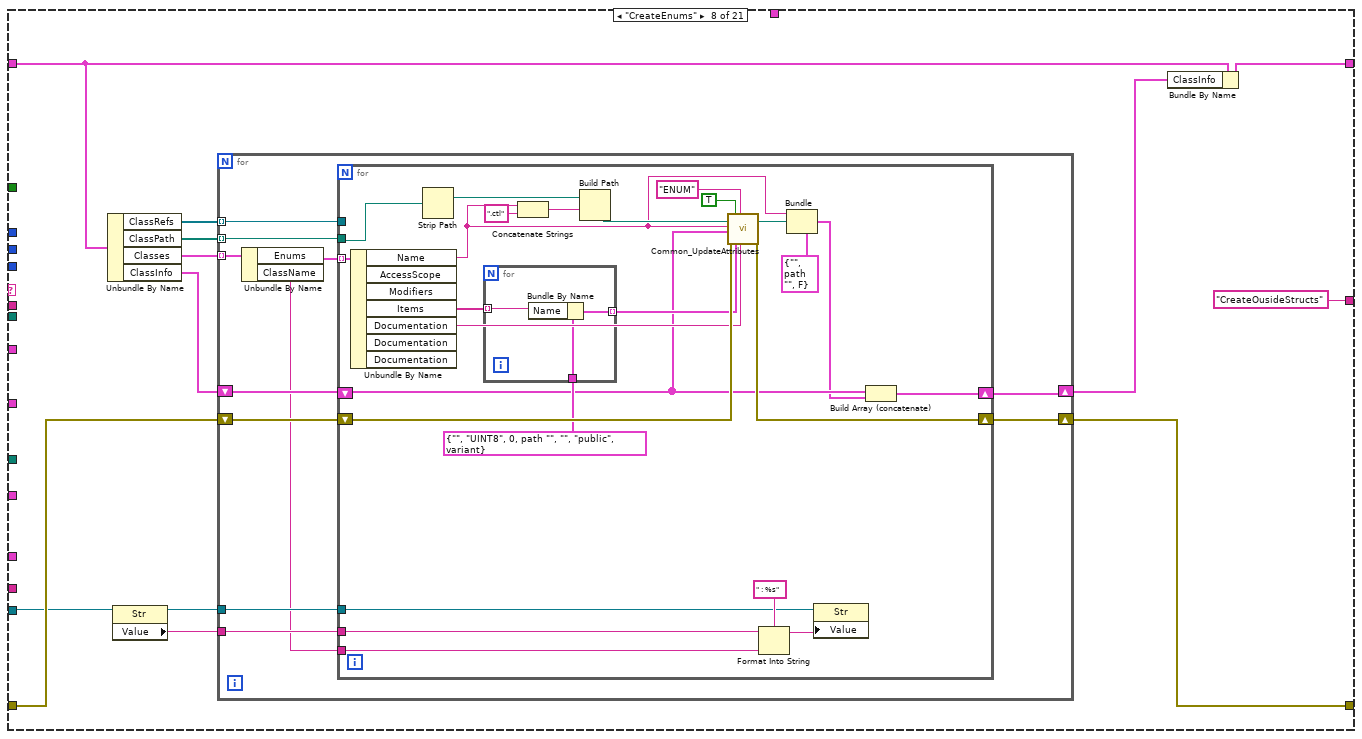
[diagram p20: hidden frame]
diagram:
  w15 = T5[] [enum."Cluster", enum."TypeDef", enum."LabVIEW Class", enum."Other", enum."ENUM"] items=["UINT8", "INT8", "UINT16", "INT16", "UINT32", "INT32", "UINT64", "INT64", "SGL", "DBL", "EXT", "CSG", "CDB", "CXT", "TimeStamp", "STRING", "PATH", "BOOL", "ENUM", "RefNum", "VIRefNum", "LabVIEW Class", "Cluster", "Variant", "TypeDef", "Waveform", "LabVIEW Object", "Other", "void", "Set", "Map"]
  w10 = "Init"
  # "If\nSystem.out.print...\nor\nConsole.Write\nThen add the Console Singleton class to the project"
  n1 = Unbundle By Name("Options") -> ("Pattern type"=w9:T10, "ClassProvider"=w12:T8, "PropertyMethodType"=w11:T9)
  n2 = disable-structure shown="Disabled" {
    frame Disabled {
      n3 = call "GDSAPI_SetClassOptions.vi"("SetAction(Set All)"=GDSAPI_SetClassOptionsAction."Set Project Icon Type", "ProjectIconType"=GDSAPI_ProjectIconType."InterfaceBlue") -> ("ProjectIcon-Before"=w22:T22)  [unwired: 6 in, 3 out]
      n4 = call "GDSAPI_SetClassOptions.vi"("SetAction(Set All)"=GDSAPI_SetClassOptionsAction."Set Project Icon Type", "ProjectIconType"=w22) -> ()  [unwired: 6 in, 4 out]
    }
    frame Enabled {
    }
  }
  n5 = while {
    shift-right: [w57] -> w20
    shift-left: "error in (no error)" -> [w58]
    shift-right: [w55] -> _
    shift-left: w10 -> [w40]
    tunnel: "TopFolder" -> [w51]
    tunnel: T21 {"App"=refnum, "Proj"=refnum, "ClassesToCreate"=[], "StructsToCreate"=[], "EnumsToCreate"=[], "Classes"=[], "ProjItem"=refnum, "ClassPath"=[], "ExistingClasses/Types"=[], "ClassRefs"=[], "ClassInfo"=[], "StartTime"=timestamp(0 s since 1904-01-01), "MissingTypes"=[], "Pattern-Before"=0, "ClassesStart"=[{"ClassName"="Program", "AccessScope"=enum."public", "Modifiers"=[], "ClassDocumentation"="", "Methods"=[{"ReturnType"={"Name"="", "DataType"=enum."void", "ArrayDim"=0, "CtrlPath"=path "", "DataTypeString"="void", "AccessScope"=enum."public", "InitialData"=variant(string "")}, "MethodName"="Main", "AccessScope"=enum."public", "Modifiers"=[enum."static"], "MethodDocumentation"="", "MethodContent"="public static void Main(string[] args)\n        {\n            // Create a subject and the observable, inject the subject into the observable\n            Subject subject = new Subject();\n            SubjectObservable observable = new SubjectObservable(subject);\n\n            //Create two observers\n            SubjectObserver zeus = new SubjectObserver(observable, \"Zeus\");\n            SubjectObserver ares = new SubjectObserver(observable, \"Ares\");\n            \n            // Run a loop and trigger the observer\n            for (int i = 0; i < 5; i++)\n            {\n                Console.WriteLine(\"Counter: \" + subject.Counter);\n                observable.inspectSubject();\n\n            }\n\n            Console.ReadLine();\n        }", "MethodArguments"=[{"Name"="args", "DataType"=enum."STRING", "ArrayDim"=1, "CtrlPath"=path "", "DataTypeString"="string[]", "AccessScope"=enum."public", "InitialData"=variant(string "")}], "GetProperty"={"Active"=FALSE, "AccessScope"=enum."public", "Code"=""}, "SetProperty"={"Active"=FALSE, "AccessScope"=enum."public", "Code"=""}}], "ParentClasses"=[], "ClassType"=enum."Class", "Owner"="Test", "OwnerType"=enum."Package/NameSpace", "Generics"=[], "Attributes"=[{"Name"="MyUINT8", "DataType"=enum."UINT8", "ArrayDim"=0, "CtrlPath"=path "", "DataTypeString"="", "AccessScope"=enum."public", "InitialData"=variant}], "Enums"=[{"Name"="MyEnum", "AccessScope"=enum."public", "Modifiers"=[], "Items"=["A1", "A2"], "Documentation"="My Enum Doc"}], "Structs"=[{"Name"="MyStruct", "AccessScope"=enum."public", "Modifiers"=[], "Items"=[{"Name"="MyObject", "DataType"=enum."LabVIEW Class", "ArrayDim"=1, "CtrlPath"=path "", "DataTypeString"="Program", "AccessScope"=enum."public", "InitialData"=variant}, {"Name"="Sträng", "DataType"=enum."STRING", "ArrayDim"=0, "CtrlPath"=path "", "DataTypeString"="", "AccessScope"=enum."public", "InitialData"=variant}], "Documentation"="Struct Doc"}]}, {"ClassName"="Subject", "AccessScope"=enum."public", "Modifiers"=[], "ClassDocumentation"="Class Subject - It has a counter object that increases everytime you inspect it", "Methods"=[{"ReturnType"={"Name"="", "DataType"=enum."INT32", "ArrayDim"=0, "CtrlPath"=path "", "DataTypeString"="int", "AccessScope"=enum."public", "InitialData"=variant(string "")}, "MethodName"="Counter", "AccessScope"=enum."public", "Modifiers"=[], "MethodDocumentation"="", "MethodContent"="public int Counter\n        {\n            get\n            {\n                return ++_counter;\n            }\n        }", "MethodArguments"=[], "GetProperty"={"Active"=TRUE, "AccessScope"=enum."public", "Code"="return ++_counter;"}, "SetProperty"={"Active"=FALSE, "AccessScope"=enum."public", "Code"=""}}], "ParentClasses"=[], "ClassType"=enum."Class", "Owner"="Test", "OwnerType"=enum."Package/NameSpace", "Generics"=[], "Attributes"=[{"Name"="_counter", "DataType"=enum."INT32", "ArrayDim"=0, "CtrlPath"=path "", "DataTypeString"="int", "AccessScope"=enum."private", "InitialData"=variant(string "")}], "Enums"=[], "Structs"=[]}, {"ClassName"="SubjectObservable", "AccessScope"=enum."public", "Modifiers"=[], "ClassDocumentation"="Class Subject Observable - The observable object that observes the subject and notifies the observers", "Methods"=[{"ReturnType"={"Name"="", "DataType"=enum."LabVIEW Object", "ArrayDim"=0, "CtrlPath"=path "", "DataTypeString"="SubjectObservable", "AccessScope"=enum."public", "InitialData"=variant(string "")}, "MethodName"="SubjectObservable", "AccessScope"=enum."public", "Modifiers"=[], "MethodDocumentation"="Accept a subject instance which we shall observe", "MethodContent"="public SubjectObservable(Subject subject)\n        {\n            _subjectObservers = new List<IObserver<Subject>>();\n            _subject = subject;\n\n        }", "MethodArguments"=[{"Name"="subject", "DataType"=enum."LabVIEW Object", "ArrayDim"=0, "CtrlPath"=path "", "DataTypeString"="Subject", "AccessScope"=enum."public", "InitialData"=variant(string "")}], "GetProperty"={"Active"=FALSE, "AccessScope"=enum."public", "Code"=""}, "SetProperty"={"Active"=FALSE, "AccessScope"=enum."public", "Code"=""}}, {"ReturnType"={"Name"="", "DataType"=enum."Other", "ArrayDim"=0, "CtrlPath"=path "", "DataTypeString"="IDisposable", "AccessScope"=enum."public", "InitialData"=variant(string "")}, "MethodName"="Subscribe", "AccessScope"=enum."public", "Modifiers"=[], "MethodDocumentation"="This method allows the observers to attach themselves. It returns a disposer object to the observer\nwhich the observer can utilize to unsubscribe", "MethodContent"="public IDisposable Subscribe(IObserver<Subject> observer)\n        {\n            if (!_subjectObservers.Contains(observer))\n            {\n                _subjectObservers.Add(observer);\n            }\n\n            return new Disposer(_subjectObservers, observer);\n        }", "MethodArguments"=[{"Name"="observer", "DataType"=enum."Other", "ArrayDim"=0, "CtrlPath"=path "", "DataTypeString"="IObserver<Subject>", "AccessScope"=enum."public", "InitialData"=variant(string "")}], "GetProperty"={"Active"=FALSE, "AccessScope"=enum."public", "Code"=""}, "SetProperty"={"Active"=FALSE, "AccessScope"=enum."public", "Code"=""}}, {"ReturnType"={"Name"="", "DataType"=enum."void", "ArrayDim"=0, "CtrlPath"=path "", "DataTypeString"="void", "AccessScope"=enum."public", "InitialData"=variant(string "")}, "MethodName"="inspectSubject", "AccessScope"=enum."public", "Modifiers"=[enum."event"], "MethodDocumentation"="This method is used to inspect the subject over time. Usually used with a timer or an event", "MethodContent"="event\n        public void inspectSubject()\n        {\n            foreach (IObserver<Subject> observer in _subjectObservers)\n            {\n                observer.OnNext(_subject);\n            }\n        }", "MethodArguments"=[], "GetProperty"={"Active"=FALSE, "AccessScope"=enum."public", "Code"=""}, "SetProperty"={"Active"=FALSE, "AccessScope"=enum."public", "Code"=""}}], "ParentClasses"=[{"ClassName"="IObservable", "ClassType"=enum."Undefined"}], "ClassType"=enum."Class", "Owner"="Test", "OwnerType"=enum."Package/NameSpace", "Generics"=["Subject"], "Attributes"=[{"Name"="_subjectObservers", "DataType"=enum."Other", "ArrayDim"=1, "CtrlPath"=path "", "DataTypeString"="IObserver<Subject>", "AccessScope"=enum."private", "InitialData"=variant(string "")}, {"Name"="_subject", "DataType"=enum."LabVIEW Object", "ArrayDim"=0, "CtrlPath"=path "", "DataTypeString"="Subject", "AccessScope"=enum."private", "InitialData"=variant(string "")}], "Enums"=[], "Structs"=[]}, {"ClassName"="SubjectObserver", "AccessScope"=enum."public", "Modifiers"=[], "ClassDocumentation"="Class Subject Observer - The object that attaches itself to a observable and recieves notifications", "Methods"=[{"ReturnType"={"Name"="", "DataType"=enum."LabVIEW Object", "ArrayDim"=0, "CtrlPath"=path "", "DataTypeString"="SubjectObserver", "AccessScope"=enum."public", "InitialData"=variant(string "")}, "MethodName"="SubjectObserver", "AccessScope"=enum."public", "Modifiers"=[], "MethodDocumentation"="", "MethodContent"="public SubjectObserver(IObservable<Subject> provider, string instanceName)\n        {\n            if (provider != null)\n            {\n                _disposer = provider.Subscribe(this);\n                _instaceName = instanceName;\n            }\n        }", "MethodArguments"=[{"Name"="provider", "DataType"=enum."Other", "ArrayDim"=0, "CtrlPath"=path "", "DataTypeString"="IObservable<Subject>", "AccessScope"=enum."public", "InitialData"=variant(string "")}, {"Name"="instanceName", "DataType"=enum."STRING", "ArrayDim"=0, "CtrlPath"=path "", "DataTypeString"="string", "AccessScope"=enum."public", "InitialData"=variant(string "")}], "GetProperty"={"Active"=FALSE, "AccessScope"=enum."public", "Code"=""}, "SetProperty"={"Active"=FALSE, "AccessScope"=enum."public", "Code"=""}}, {"ReturnType"={"Name"="", "DataType"=enum."void", "ArrayDim"=0, "CtrlPath"=path "", "DataTypeString"="void", "AccessScope"=enum."public", "InitialData"=variant(string "")}, "MethodName"="OnNext", "AccessScope"=enum."public", "Modifiers"=[], "MethodDocumentation"="The observable invokes this method to pass the Subject object to the observer", "MethodContent"="public void OnNext(Subject value)\n        {\n            Console.WriteLine(\"[\" + _instaceName + \"] \" + value.Counter);\n        }", "MethodArguments"=[{"Name"="value", "DataType"=enum."LabVIEW Object", "ArrayDim"=0, "CtrlPath"=path "", "DataTypeString"="Subject", "AccessScope"=enum."public", "InitialData"=variant(string "")}], "GetProperty"={"Active"=FALSE, "AccessScope"=enum."public", "Code"=""}, "SetProperty"={"Active"=FALSE, "AccessScope"=enum."public", "Code"=""}}, {"ReturnType"={"Name"="", "DataType"=enum."void", "ArrayDim"=0, "CtrlPath"=path "", "DataTypeString"="void", "AccessScope"=enum."public", "InitialData"=variant(string "")}, "MethodName"="OnCompleted", "AccessScope"=enum."public", "Modifiers"=[], "MethodDocumentation"="Usually called when a transmission is complete. Not implemented.", "MethodContent"="public void OnCompleted()\n        {\n            throw new NotImplementedException();\n        }", "MethodArguments"=[], "GetProperty"={"Active"=FALSE, "AccessScope"=enum."public", "Code"=""}, "SetProperty"={"Active"=FALSE, "AccessScope"=enum."public", "Code"=""}}, {"ReturnType"={"Name"="", "DataType"=enum."void", "ArrayDim"=0, "CtrlPath"=path "", "DataTypeString"="void", "AccessScope"=enum."public", "InitialData"=variant(string "")}, "MethodName"="OnError", "AccessScope"=enum."public", "Modifiers"=[], "MethodDocumentation"="Usually called when there was an error. Didn't implement.", "MethodContent"="public void OnError(Exception error)\n        {\n            throw new NotImplementedException();\n        }", "MethodArguments"=[{"Name"="error", "DataType"=enum."Other", "ArrayDim"=0, "CtrlPath"=path "", "DataTypeString"="Exception", "AccessScope"=enum."public", "InitialData"=variant(string "")}], "GetProperty"={"Active"=FALSE, "AccessScope"=enum."public", "Code"=""}, "SetProperty"={"Active"=FALSE, "AccessScope"=enum."public", "Code"=""}}, {"ReturnType"={"Name"="", "DataType"=enum."void", "ArrayDim"=0, "CtrlPath"=path "", "DataTypeString"="void", "AccessScope"=enum."public", "InitialData"=variant(string "")}, "MethodName"="Dispose", "AccessScope"=enum."public", "Modifiers"=[], "MethodDocumentation"="Invoke the disposer recieved from the observable. This will unsubscribe", "MethodContent"="public void Dispose()\n        {\n            _disposer.Dispose();\n        }", "MethodArguments"=[], "GetProperty"={"Active"=FALSE, "AccessScope"=enum."public", "Code"=""}, "SetProperty"={"Active"=FALSE, "AccessScope"=enum."public", "Code"=""}}], "ParentClasses"=[{"ClassName"="IObserver", "ClassType"=enum."Undefined"}], "ClassType"=enum."Class", "Owner"="Test", "OwnerType"=enum."Package/NameSpace", "Generics"=["Subject"], "Attributes"=[{"Name"="_disposer", "DataType"=enum."Other", "ArrayDim"=0, "CtrlPath"=path "", "DataTypeString"="IDisposable", "AccessScope"=enum."private", "InitialData"=variant(string "")}, {"Name"="_instaceName", "DataType"=enum."STRING", "ArrayDim"=0, "CtrlPath"=path "", "DataTypeString"="string", "AccessScope"=enum."private", "InitialData"=variant(string "")}], "Enums"=[], "Structs"=[]}, {"ClassName"="Disposer", "AccessScope"=enum."private", "Modifiers"=[], "ClassDocumentation"="Private class Disposer: Implements the IDisposable. Observable returns an instance to the observer for easy unsubscription\nprivate", "Methods"=[{"ReturnType"={"Name"="", "DataType"=enum."LabVIEW Object", "ArrayDim"=0, "CtrlPath"=path "", "DataTypeString"="Disposer", "AccessScope"=enum."public", "InitialData"=variant(string "")}, "MethodName"="Disposer", "AccessScope"=enum."public", "Modifiers"=[], "MethodDocumentation"="", "MethodContent"="public Disposer(List<IObserver<Subject>> _subObservers, IObserver<Subject> observer)\n            {\n                _subjectObservers = _subObservers;\n                _observer = observer;\n            }", "MethodArguments"=[{"Name"="_subObservers", "DataType"=enum."Other", "ArrayDim"=1, "CtrlPath"=path "", "DataTypeString"="IObserver<Subject>", "AccessScope"=enum."public", "InitialData"=variant(string "")}, {"Name"="observer", "DataType"=enum."Other", "ArrayDim"=0, "CtrlPath"=path "", "DataTypeString"="IObserver<Subject>", "AccessScope"=enum."public", "InitialData"=variant(string "")}], "GetProperty"={"Active"=FALSE, "AccessScope"=enum."public", "Code"=""}, "SetProperty"={"Active"=FALSE, "AccessScope"=enum."public", "Code"=""}}, {"ReturnType"={"Name"="", "DataType"=enum."void", "ArrayDim"=0, "CtrlPath"=path "", "DataTypeString"="void", "AccessScope"=enum."public", "InitialData"=variant(string "")}, "MethodName"="Dispose", "AccessScope"=enum."public", "Modifiers"=[], "MethodDocumentation"="", "MethodContent"="public void Dispose()\n            {\n                if (_subjectObservers.Contains(_observer))\n                {\n                    _subjectObservers.Remove(_observer);\n                }\n            }", "MethodArguments"=[], "GetProperty"={"Active"=FALSE, "AccessScope"=enum."public", "Code"=""}, "SetProperty"={"Active"=FALSE, "AccessScope"=enum."public", "Code"=""}}], "ParentClasses"=[{"ClassName"="IDisposable", "ClassType"=enum."Undefined"}], "ClassType"=enum."Class", "Owner"="SubjectObservable", "OwnerType"=enum."Class", "Generics"=[], "Attributes"=[{"Name"="_subjectObservers", "DataType"=enum."Other", "ArrayDim"=1, "CtrlPath"=path "", "DataTypeString"="IObserver<Subject>", "AccessScope"=enum."private", "InitialData"=variant(string "")}, {"Name"="_observer", "DataType"=enum."Other", "ArrayDim"=0, "CtrlPath"=path "", "DataTypeString"="IObserver<Subject>", "AccessScope"=enum."private", "InitialData"=variant(string "")}], "Enums"=[], "Structs"=[]}]} -> [w50]
    shift-right: [w35] -> w6
    shift-left: _ -> [w49]
    tunnel: "Classes" -> [w48]
    tunnel: "MissingItems" -> [w32]
    tunnel: w15 -> [w47]
    tunnel: w12 -> [w46]
    tunnel: "ExistingClassFolders" -> [w45]
    tunnel: "ProgressTextRef" -> [w44]
    tunnel: "ProgressTextRef" -> [w36]
    tunnel: w11 -> [w34]
    shift-left: w10 -> [w33]
    tunnel: w9 -> [w31]
    tunnel: "EnumsOusideClass" -> [w29]
    tunnel: "StructsOusideClass" -> [w28]
    tunnel: "InterfacesThatShouldBeConvertedToClasses" -> [w27]
    tunnel: "BetterNames" -> [w26]
    i -> [w42]
    stop <- w52 stop-if-true
    n6 = property class="Str"(reference=w44) -> (reference out=w43:refnum<vi>, "Value"=w39:string)  [unwired: 1 in, 1 out]
    n7 = case shown="Default" w42 {
      tunnel: [w59 w61] -> w41
      tunnel: w40 -> [w59 w62]
      tunnel: w39 -> [_ w63]
      frame 0 {
      }
      frame Default {
        n8 = Concatenate Strings(w63, "\n" ("string"), w62) -> (w61:string)
      }
    }
    n9 = property class="Str"(reference=w43, "Value"=w41, "Text.Scroll Position"=u32 4294967295) -> (error out=w37:errorcluster)  [unwired: 1 in, 1 out]
    n10 = case shown="\"CreateMethods\"" w40 {
      tunnel: w58 -> [w74 w142 w225 w310 w335 w361 w402 w509 w564 w595 w644 w691 w725 w756 w811 w876 w901 w929 w972 w1001 w1012]
      tunnel: [w79 w142 w225 w310 w326 w360 w401 w508 w563 w594 w643 w691 w725 w755 w810 w875 w900 w929 w972 w1000 w1011] -> w57
      tunnel: ["SortClasses" "SortStructs" "OrderClasses" "CreateProject" "CreateOutsideEnums" "CreateClasses" "CreateEnums" "CreateOusideStructs" "CreateStruct" "UpdateAttribute" "UpdateParentClassTypes" "UpdateMethodTypes" "UpdateConstructors" "UpdateDestructors" "AddInterfaceMethods" "CreateMethods" "AddExtraClasses?" "SaveAll" "Done" "CloseDown" "Exit"] -> w54
      tunnel: w51 -> [_ _ _ _ w319 w357 _ _ w557 _ _ _ _ _ _ _ _ w925 _ _ _]
      tunnel: w50 -> [w87 _ _ _ _ _ _ _ _ _ _ _ _ _ _ _ _ _ _ _ _]
      tunnel: [w86 w139 w222 w300 w331 w354 w399 w511 w566 w597 w638 w692 w726 w760 w815 w874 w899 w924 w971 w1009 w1014] -> w35
      tunnel: w49 -> [_ w141 w224 w308 w332 w355 w407 w516 w568 w602 w645 w690 w724 w759 w814 w874 w899 w924 w971 w1009 w1014]
      tunnel: w48 -> [w66 _ _ _ _ _ _ _ _ _ _ _ _ _ _ _ _ w927 _ _ _]
      tunnel: w32 -> [w85 _ _ _ _ _ _ _ _ _ _ _ _ _ _ _ _ _ _ _ _]
      tunnel: w47 -> [_ w136 w221 _ _ _ _ _ _ _ _ _ _ _ _ _ _ _ _ _ _]
      tunnel: w46 -> [_ _ _ _ _ _ w405 _ _ _ _ _ _ _ _ _ _ _ _ _ _]
      tunnel: w45 -> [w78 _ _ _ _ _ _ _ _ _ _ _ _ _ _ _ _ _ _ _ _]
      tunnel: w37 -> [_ _ _ _ _ _ _ _ _ _ _ _ _ _ _ _ _ _ _ _ _]
      tunnel: w36 -> [_ _ _ _ _ w359 w395 w507 w562 w592 w641 _ _ _ _ w873 w898 _ _ w990 _]
      tunnel: w34 -> [_ _ _ _ _ _ _ _ _ _ _ _ _ _ _ _ w895 _ _ _ _]
      tunnel: w33 -> [_ _ _ _ _ _ _ _ _ _ _ _ _ _ _ _ _ _ _ _ _]
      tunnel: w31 -> [w73 _ _ _ _ _ _ _ _ _ _ _ _ _ _ _ _ _ _ _ _]
      tunnel: w29 -> [_ _ _ _ _ w358 _ _ _ _ _ _ _ _ _ _ _ _ _ _ _]
      tunnel: w28 -> [_ _ _ _ _ _ _ _ w558 _ _ _ _ _ _ _ _ _ _ _ _]
      tunnel: w27 -> [w70 _ _ _ _ _ _ _ _ _ _ _ _ _ _ _ _ _ _ _ _]
      tunnel: w26 -> [w64 _ _ _ _ _ _ _ _ _ _ _ _ _ _ _ _ _ _ _ _]
      frame "Init" {
        # "Interfaces are now supported"
        n11 = case shown="True" w64 {
          tunnel: w66 -> [w95 w97]
          tunnel: [w95 w96] -> w65
          frame False {
          }
          frame True {
            n12 = call "ConvertTextBasedCodeToLabVIEW_MakenamesBetter.vi"("ClassesIn"=w97) -> ("ClassesOut"=w96:T11[])  [unwired: 10 in]
          }
        }
        n13 = call "GDSAPI_SetClassOptions.vi"("SetAction(Set All)"=GDSAPI_SetClassOptionsAction."Set Pattern Type", "error in (no error)"=w74, "PatternIn"=w73) -> ("error out"=w68:errorcluster, "Pattern-Before"=w71:T10)  [unwired: 5 in, 2 out]
        n14 = for {
          tunnel: w65 -> [w113] mode=indexing
          tunnel: [w110] -> w84 mode=concatenating
          n15 = Unbundle By Name(w113) -> ("ClassName"=w111:string, "Enums"=w112:T6[])
          n16 = for {
            tunnel: w112 -> [w118] mode=indexing
            tunnel: w111 -> [w115]
            tunnel: [w114] -> w110 mode=indexing
            n17 = Unbundle By Name(w118) -> ("Name"=w116:string)
            n18 = Concatenate Strings(w115, ":#:" ("string"), w116) -> (w114:string)
          }
        }
        n19 = for {
          tunnel: w85 -> [w130] mode=indexing
          tunnel: [w120] -> w82 mode=indexing if=w121
          tunnel: [w122] -> w81 mode=indexing if=w121
          tunnel: [w120] -> w75 mode=indexing if=w119
          n20 = Unbundle By Name(w130) -> ("Item"=w120:string, "Icons"=w129:T18[], "Index"=w125:i32, "Options"=w126:string[])
          n21 = Index Array(array=w129, index=w125) -> (element=w128:T18)
          n22 = Index Array(array=w126, index=w125) -> (element=w124:string)
          n23 = Scan From String(input string=w124, default 1=ConvertTextBasedCodeToLabVIEW_MissingTypeOptions."Create stub code as class") -> (output 1=w122:T23)  [unwired: 3 in, 3 out]
          n24 = Equal?(x=w128, y=ConvertTextBasedCodeToLabVIEW_MissingTypeIconType."Add") -> (x = y?=w121:bool)
          n25 = Not(x=w121) -> (.not. x?=w119:bool)
        }
        n26 = for {
          tunnel: w78 -> [w99] mode=indexing
          tunnel: [w98] -> w77 mode=concatenating
          n27 = call <vilib>:"Recursive File List.vi"("pattern"="*.lvclass", "Folder Path"=w99) -> ("All Files in Dir"=w103:path[])  [unwired: 5 in, 4 out]
          n28 = call <vilib>:"Recursive File List.vi"("pattern"="*.ctl", "Folder Path"=w99) -> ("All Files in Dir"=w102:path[])  [unwired: 5 in, 4 out]
          n29 = for {
            tunnel: w103 -> [w109] mode=indexing
            tunnel: [w108] -> w101 mode=indexing
            n30 = call <vilib>:"Get File Extension.vi"("file"=w109) -> ("filename without extension"=w108:string)  [unwired: 6 in, 4 out]
          }
          n31 = for {
            tunnel: w102 -> [w107] mode=indexing
            tunnel: [w106] -> w100 mode=indexing
            n32 = call <vilib>:"Get File Extension.vi"("file"=w107) -> ("filename without extension"=w106:string)  [unwired: 6 in, 4 out]
          }
          n33 = Build Array (concatenate)(w101, w100) -> (w98:string[])
        }
        n34 = disable-structure shown="Enabled" {
          disable-tunnel: w70 -> [w92 _]
          disable-tunnel: [w91 w94] -> w69
          disable-tunnel: w68 -> [w90 w93]
          disable-tunnel: [w89 w93] -> w67
          disable-tunnel: w65 -> [w88 w94]
          frame Disabled {
            n35 = call "ConvertTextBasedCodeToLabVIEW_ChangeInterfaceToInheritace.vi"("error in (no error)"=w90, "InterfacesThatShouldBeConvertedToClasses"=w92, "ClassesIn"=w88) -> ("error out"=w89:errorcluster, "ClassesOut"=w91:T11[])  [unwired: 7 in]
          }
          frame Enabled {
          }
        }
        n36 = call "ConvertTextBasedCodeToLabVIEW_CreateMissingClassesDefinition.vi"("error in (no error)"=w67, "Action"=w81, "ClassName"=w82) -> ("error out"=w79:errorcluster, "Classes"=w80:T11[])  [unwired: 7 in]
        n37 = Get Date/Time In Seconds() -> (seconds since 1Jan1904=w76:timestamp)
        n38 = Bundle By Name(cluster=w87, "StartTime"=w76, "EnumsToCreate"=w84, "MissingTypes"=w75, "ClassesToCreate"=w82, "Classes"=w80, "ExistingClasses/Types"=w77, "Pattern-Before"=w71, "ClassesStart"=w69) -> (w86:T21)
      }
      frame "SortClasses" {
        n39 = Unbundle By Name(w141) -> ("ExistingClasses/Types"=w138:string[], "ClassesToCreate"=w140:string[], "ClassesStart"=w131:T11[])
        n40 = To Lower Case(string=w138) -> (all lower case string=w137:string[])
        n41 = while {
          shift-right: [w155] -> w135
          shift-left: w140 -> [w156]
          shift-right: [w153] -> w133
          shift-left: w131 -> [w152]
          tunnel: w137 -> [w147]
          tunnel: w136 -> [w146]
          stop <- w148 stop-if-true
          n42 = for {
            tunnel: w152 -> [w157] mode=indexing
            shift-right: [w167] -> w155
            shift-left: w156 -> [w165]
            tunnel: [w157] -> w153 mode=indexing if=w166
            tunnel: w147 -> [w162]
            tunnel: w146 -> [w164]
            n43 = Unbundle By Name(w157) -> ("ClassName"=w168:string, "ParentClasses"=w171:T14[], "Attributes"=w163:T4[])
            n44 = To Lower Case(string=w165) -> (all lower case string=w161:string[])
            n45 = disable-structure shown="Enabled" {
              disable-tunnel: w164 -> [w182 _]
              disable-tunnel: w163 -> [w180 _]
              disable-tunnel: w162 -> [w179 _]
              disable-tunnel: w161 -> [w178 _]
              disable-tunnel: [w173 TRUE] -> w159
              frame Disabled {
                n46 = for {
                  tunnel: w180 -> [w195] mode=indexing
                  tunnel: w182 -> [w194]
                  tunnel: [w191] -> w174 mode=indexing if=w192
                  n47 = Unbundle By Name(w195) -> ("DataType"=w193:T5, "DataTypeString"=w191:string)
                  n48 = Search 1D Array(1D array=w194, element=w193) -> (index of element=w196:i32)  [unwired: 1 in]
                  n49 = Greater Or Equal To 0?(x=w196) -> (x >= 0?=w192:bool)
                }
                n50 = To Lower Case(string=w174) -> (all lower case string=w177:string[])
                n51 = Empty Array?(array=w174) -> (empty?=w176:bool)
                n52 = for {
                  tunnel: w178 -> [w189]
                  tunnel: [w184] -> w181 mode=indexing
                  tunnel: w179 -> [w188]
                  tunnel: w177 -> [w183] mode=indexing
                  n53 = Search 1D Array(1D array=w188, element=w183) -> (index of element=w187:i32)  [unwired: 1 in]
                  n54 = Search 1D Array(1D array=w189, element=w183) -> (index of element=w190:i32)  [unwired: 1 in]
                  n55 = Greater Or Equal To 0?(x=w187) -> (x >= 0?=w185:bool)
                  n56 = Greater Or Equal To 0?(x=w190) -> (x >= 0?=w186:bool)
                  n57 = Or(x=w185, y=w186) -> (x .or. y?=w184:bool)
                }
                n58 = And Array Elements(Boolean array=w181) -> (logical AND=w175:bool)
                n59 = Or(x=w175, y=w176) -> (x .or. y?=w173:bool)
              }
              frame Enabled {
              }
            }
            n60 = for {
              tunnel: w171 -> [w211] mode=indexing
              tunnel: w161 -> [w209]
              tunnel: [w202] -> w172 mode=indexing
              tunnel: w162 -> [w208]
              n61 = Unbundle By Name(w211) -> ("ClassName"=w207:string)
              n62 = To Lower Case(string=w207) -> (all lower case string=w206:string)
              n63 = Search 1D Array(1D array=w208, element=w206) -> (index of element=w205:i32)  [unwired: 1 in]
              n64 = Search 1D Array(1D array=w209, element=w206) -> (index of element=w210:i32)  [unwired: 1 in]
              n65 = Greater Or Equal To 0?(x=w205) -> (x >= 0?=w203:bool)
              n66 = Greater Or Equal To 0?(x=w210) -> (x >= 0?=w204:bool)
              n67 = Or(x=w203, y=w204) -> (x .or. y?=w202:bool)
            }
            n68 = Empty Array?(array=w171) -> (empty?=w169:bool)
            n69 = And Array Elements(Boolean array=w172) -> (logical AND=w170:bool)
            n70 = Or(x=w170, y=w169) -> (x .or. y?=w160:bool)
            n71 = Compound Arithmetic op=AND(w160, w159) -> (w158:bool)
            n72 = Not(x=w158) -> (.not. x?=w166:bool)
            n73 = case shown="True" w158 {
              tunnel: w165 -> [w198 w201]
              tunnel: w168 -> [_ w200]
              tunnel: [w198 w199] -> w167
              frame False {
              }
              frame True {
                n74 = Build Array (concatenate)(w201, w200) -> (w199:string[])
              }
            }
          }
          n75 = Array Size(array=w153) -> (size(s)=w151:i32)
          n76 = Array Size(array=w152) -> (size(s)=w150:i32)
          n77 = Empty Array?(array=w153) -> (empty?=w154:bool)
          n78 = Equal?(x=w151, y=w150) -> (x = y?=w149:bool)
          n79 = Or(x=w154, y=w149) -> (x .or. y?=w148:bool)
        }
        n80 = for {
          tunnel: w133 -> [w145] mode=indexing
          tunnel: [w144] -> w132 mode=indexing
          n81 = Unbundle By Name(w145) -> ("ClassName"=w144:string)
        }
        n82 = Build Array (concatenate)(w135, w132) -> (w134:string[])
        n83 = Bundle By Name(cluster=w141, "ClassesToCreate"=w134) -> (w139:T21)
      }
      frame "SortStructs" {
        n84 = Unbundle By Name(w224) -> ("EnumsToCreate"=w220:string[], "ClassesToCreate"=w219:string[], "StructsToCreate"=w223:string[], "ClassesStart"=w212:T11[])
        n85 = while {
          shift-right: [w239] -> w215
          shift-left: w223 -> [w240]
          shift-right: [w232] -> w216
          shift-left: w212 -> [w238]
          tunnel: w221 -> [w235]
          tunnel: w220 -> [w234]
          tunnel: w219 -> [w233]
          shift-right: [w229] -> _
          shift-left: 0 -> [w230]
          stop <- w236 stop-if-true
          n86 = for {
            tunnel: w238 -> [w245] mode=indexing
            shift-right: [w246] -> w239
            shift-left: w240 -> [w251]
            tunnel: w235 -> [w250]
            tunnel: w234 -> [w248]
            tunnel: w233 -> [w247]
            tunnel: [w242] -> w231 mode=indexing
            tunnel: [w244] -> w232 mode=indexing
            n87 = Unbundle By Name(w245) -> ("ClassName"=w249:string, "Structs"=w243:T1[])
            n88 = for {
              tunnel: w243 -> [w254] mode=indexing
              tunnel: w249 -> [w264]
              shift-right: [w256] -> w246
              shift-left: w251 -> [w257]
              tunnel: w250 -> [w269]
              tunnel: w248 -> [w266]
              tunnel: w247 -> [w262]
              tunnel: [w254] -> w241 mode=indexing if=w252
              n89 = Unbundle By Name(w254) -> ("Name"=w263:string, "Items"=w270:T4[])
              n90 = Concatenate Strings(w264, ":#:" ("string"), w263) -> (w255:string)
              n91 = for {
                tunnel: w266 -> [w277] mode=indexing
                tunnel: [w275] -> w261 mode=indexing
                n92 = Match Pattern(string=w277, regular expression=":#:" ("string")) -> (after substring=w275:string)  [unwired: 1 in, 3 out]
              }
              n93 = for {
                tunnel: w257 -> [w280] mode=indexing
                tunnel: [w278] -> w267 mode=indexing
                n94 = Match Pattern(string=w280, regular expression=":#:" ("string")) -> (after substring=w278:string)  [unwired: 1 in, 3 out]
              }
              n95 = for {
                tunnel: w270 -> [w296] mode=indexing
                tunnel: w269 -> [w295]
                tunnel: [w292] -> w268 mode=indexing if=w293
                n96 = Unbundle By Name(w296) -> ("DataType"=w294:T5, "DataTypeString"=w292:string)
                n97 = Search 1D Array(1D array=w295, element=w294) -> (index of element=w297:i32)  [unwired: 1 in]
                n98 = Greater Or Equal To 0?(x=w297) -> (x >= 0?=w293:bool)
              }
              n99 = Empty Array?(array=w268) -> (empty?=w258:bool)
              n100 = for {
                tunnel: w267 -> [w291]
                tunnel: w268 -> [w288] mode=indexing
                tunnel: w262 -> [w290]
                tunnel: w261 -> [w289]
                tunnel: [w281] -> w260 mode=indexing
                n101 = Search 1D Array(1D array=w289, element=w288) -> (index of element=w285:i32)  [unwired: 1 in]
                n102 = Search 1D Array(1D array=w290, element=w288) -> (index of element=w286:i32)  [unwired: 1 in]
                n103 = Search 1D Array(1D array=w291, element=w288) -> (index of element=w287:i32)  [unwired: 1 in]
                n104 = Greater Or Equal To 0?(x=w285) -> (x >= 0?=w283:bool)
                n105 = Greater Or Equal To 0?(x=w286) -> (x >= 0?=w284:bool)
                n106 = Greater Or Equal To 0?(x=w287) -> (x >= 0?=w282:bool)
                n107 = Compound Arithmetic op=OR(w283, w284, w282) -> (w281:bool)
              }
              n108 = And Array Elements(Boolean array=w260) -> (logical AND=w259:bool)
              n109 = Or(x=w259, y=w258) -> (x .or. y?=w253:bool)
              n110 = case shown="True" w253 {
                tunnel: [w271 w274] -> w256
                tunnel: w257 -> [w271 w273]
                tunnel: w255 -> [_ w272]
                frame False {
                }
                frame True {
                  n111 = Build Array (concatenate)(w273, w272) -> (w274:string[])
                }
              }
              n112 = Not(x=w253) -> (.not. x?=w252:bool)
            }
            n113 = Bundle By Name(cluster=w245, "Structs"=w241) -> (w244:T11)
            n114 = Array Size(array=w241) -> (size(s)=w242:i32)
          }
          n115 = Add Array Elements(numeric array=w231) -> (sum=w229:i32)
          n116 = Equal?(x=w229, y=w230) -> (x = y?=w237:bool)
          n117 = Equal To 0?(x=w229) -> (x = 0?=w228:bool)
          n118 = Or(x=w228, y=w237) -> (x .or. y?=w236:bool)
        }
        n119 = for {
          tunnel: w216 -> [w227] mode=indexing
          tunnel: [w226] -> w213 mode=indexing
          n120 = Unbundle By Name(w227) -> ("ClassName"=w226:string)
        }
        n121 = Build Array (concatenate)(w215, w213) -> (w214:string[])
        n122 = Bundle By Name(cluster=w224, "StructsToCreate"=w214) -> (w222:T21)
      }
      frame "OrderClasses" {
        n123 = Unbundle By Name(w308) -> ("ClassesToCreate"=w307:string[], "Classes"=w301:T11[], "ClassesStart"=w298:T11[])  [unwired: 2 out]
        n124 = for {
          tunnel: w298 -> [w312] mode=indexing
          tunnel: [w311] -> w303 mode=indexing
          n125 = Unbundle By Name(w312) -> ("ClassName"=w311:string)
        }
        n126 = Array Size(array=w301) -> (size(s)=w306:i32)
        n127 = Delete From Array(array=w307, length=w306, index=0) -> (array with subset deleted=w304:string[])  [unwired: 1 out]
        n128 = for {
          tunnel: w304 -> [w316] mode=indexing
          tunnel: w303 -> [w317]
          tunnel: w298 -> [w315]
          tunnel: [w313] -> w302 mode=indexing
          n129 = Search 1D Array(1D array=w317, element=w316) -> (index of element=w314:i32)  [unwired: 1 in]
          n130 = Index Array(array=w315, index=w314) -> (element=w313:T11)
        }
        n131 = Build Array (concatenate)(w301, w302) -> (w299:T11[])
        n132 = Bundle By Name(cluster=w308, "Classes"=w299) -> (w300:T21)
      }
      frame "CreateProject" {
        # "Set APP Ref to use when opening VIs from now on"
        n133 = invoke class="App" method="Project.New"(error in=w335) -> (error out=w333:errorcluster, "Project:New"=w334:refnum<vi>)  [unwired: 2 in, 1 out]
        n134 = call <vilib>:"Create Directory Recursive.vi"("directory"=w319) -> ("directory copy"=w318:path)  [unwired: 4 in, 2 out]
        n135 = for {
          N: 100 -> [_]
          tunnel: w318 -> [w338]
          tunnel: w333 -> [w337]
          tunnel: [w348] -> w321
          shift-right: [w349] -> w322
          shift-left: w334 -> [w350]
          i -> [w341]
          stop <- w345 continue-if-true
          n136 = Strip Path(path=w338) -> (name=w340:string)  [unwired: 1 out]
          n137 = case shown="Default" w341 {
            selector: w341 -> [w353 _]
            tunnel: [w351 _] -> w339
            frame Default {
              n138 = Format Into String(format string="(%d)", w353) -> (resulting string=w351:string)  [unwired: 2 in, 1 out]
            }
            frame 0 {
            }
          }
          n139 = Concatenate Strings(w340, w339, ".lvproj" ("string")) -> (w344:string)
          n140 = Build Path(base path=w338, name or relative path=w344) -> (appended path=w342:path)
          n141 = invoke class="Project" method="Save"(reference=w350, error in=w337, "Path"=w342) -> (reference out=w349:refnum<vi>, error out=w348:errorcluster)  [unwired: 1 in, 2 out]
          n142 = Unbundle By Name(w348) -> ("code"=w347:i32)
          n143 = Equal?(x=1357, y=w347) -> (x = y?=w345:bool)
        }
        n144 = invoke class="Project" method="Open Window"(reference=w322, error in=w321) -> (reference out=w324:refnum<vi>, error out=w323:errorcluster)  [unwired: 1 in, 1 out]
        n145 = property class="Project"(reference=w324, error in=w323) -> (reference out=w330:refnum<vi>, error out=w329:errorcluster, "App Ref"=w325:refnum<vi>)
        n146 = property class="Project"(reference=w330, error in=w329) -> (error out=w327:errorcluster, "My Computer"=w328:refnum<vi>)  [unwired: 1 out]
        n147 = Bundle By Name(cluster=w332, "Proj"=w330, "App"=w325, "ProjItem"=w328) -> (w331:T21)
        n148 = call "CommonVIs_UmlOpenVIRef.vi"("error in"=w327, "AppRef"=w325) -> ("error out"=w326:errorcluster)  [unwired: 6 in, 3 out]
      }
      frame "CreateOutsideEnums" {
        n149 = Unbundle By Name(w355) -> ("ClassInfo"=w364:T20[])
        n150 = property class="Str"(reference=w359) -> (reference out=w363:refnum<vi>, "Value"=w362:string)  [unwired: 1 in, 1 out]
        n151 = for {
          tunnel: w358 -> [w388] mode=indexing
          shift-right: [w386] -> w360
          shift-left: w361 -> [w387]
          shift-right: [w376] -> w356
          shift-left: w364 -> [w378]
          tunnel: w363 -> [w370]
          tunnel: w362 -> [w369]
          tunnel: w357 -> [w367]
          n152 = Unbundle By Name(w388) -> ("Name"=w368:string, "Items"=w382:string[], "Documentation"=w383:string)  [unwired: 4 out]
          n153 = for {
            tunnel: w382 -> [w390] mode=indexing
            tunnel: T4 {"Name"="", "DataType"=enum."UINT8", "ArrayDim"=0, "CtrlPath"=path "", "DataTypeString"="", "AccessScope"=enum."public", "InitialData"=variant} -> [w391]
            tunnel: [w389] -> w380 mode=indexing
            n154 = Bundle By Name(cluster=w391, "Name"=w390) -> (w389:T4)
          }
          n155 = Concatenate Strings(w368, ".ctl" ("string")) -> (w374:string)
          n156 = Build Path(base path=w367, name or relative path=w374) -> (appended path=w373:path)
          n157 = call "Common_UpdateAttributes.vi"("ClassPath/LvClassRef"=w373, "NewAttributes"=w368, "ClassInfo"=w378, "error in (no error)"=w387, "Don't Prompt (False)"=TRUE, "Attributes"=w380, "Stereotype"="ENUM" ("regular expression"), "Ctl-Description"=w383) -> ("CtlPath"=w379:path, "error out"=w386:errorcluster)  [unwired: 9 in, 1 out]
          n158 = Format Into String(format string=" : %s", initial string=w369, w368) -> (resulting string=w372:string)  [unwired: 1 in, 1 out]
          n159 = Bundle(cluster=T20 {"ClassNamn"="", "ClassPath"=path "", "InterfaceClass"=FALSE} ("Cluster"), "ClassNamn"=w368, "ClassPath"=w379) -> (w377:T20)  [unwired: 1 in]
          n160 = property class="Str"(reference=w370, "Value"=w372) -> ()  [unwired: 1 in, 2 out]
          n161 = Build Array (concatenate)(w378, w377) -> (w376:T20[])
        }
        n162 = Bundle By Name(cluster=w355, "ClassInfo"=w356) -> (w354:T21)
      }
      frame "CreateClasses" {
        w403 = path[] []
        w404 = string[] []
        n163 = Unbundle By Name(w407) -> ("ProjItem"=w400:refnum<vi>, "Classes"=w406:T11[], "ClassInfo"=w392:T20[])
        n164 = property class="Str"(reference=w395) -> (reference out=w393:refnum<vi>, "Value"=w394:string)  [unwired: 1 in, 1 out]
        n165 = for {
          tunnel: w406 -> [w438] mode=indexing
          tunnel: w405 -> [w439]
          shift-right: [w436] -> _
          shift-left: w404 -> [w412]
          shift-right: [w435] -> _
          shift-left: w403 -> [w411]
          shift-right: [w433] -> _
          shift-left: w404 -> [w430]
          shift-right: [w434] -> _
          shift-left: w403 -> [w431]
          shift-right: [w429] -> w401
          shift-left: w402 -> [w413]
          tunnel: w400 -> [w428]
          tunnel: [w417] -> w398 mode=indexing
          tunnel: [w427] -> w397 mode=indexing
          tunnel: w394 -> [w424]
          tunnel: w393 -> [w422]
          shift-right: [w419] -> w396
          shift-left: w392 -> [w418]
          (unwired) TRUE
          n166 = Unbundle By Name(w438) -> ("ClassName"=w420:string, "ClassDocumentation"=w437:string, "ClassType"=w415:T15, "ParentClasses"=w425:T14[])
          n167 = for {
            tunnel: w430 -> [w450]
            tunnel: w431 -> [w449]
            tunnel: [w448] -> w432 mode=indexing if=w445
            tunnel: w425 -> [w447] mode=indexing
            tunnel: w412 -> [w443]
            tunnel: w411 -> [w442]
            tunnel: [w441] -> w410 if=w440
            n168 = Unbundle By Name(w447) -> ("ClassType"=w444:T15, "ClassName"=w446:string)
            n169 = case shown="\"Class\", Default" w444 {
              tunnel: w450 -> [_ w462]
              tunnel: w449 -> [_ w461]
              tunnel: [_ w460] -> w448
              tunnel: w446 -> [w455 w458]
              tunnel: [_ w457] -> w445
              tunnel: w443 -> [w456 _]
              tunnel: w442 -> [w454 _]
              tunnel: [w453 _] -> w441
              tunnel: [w451 _] -> w440
              frame "Class", Default {
                n170 = Search 1D Array(1D array=w456, element=w455) -> (index of element=w452:i32)  [unwired: 1 in]
                n171 = Index Array(array=w454, index=w452) -> (element=w453:path)
                n172 = Greater Or Equal To 0?(x=w452) -> (x >= 0?=w451:bool)
              }
              frame "Interface" {
                n173 = Search 1D Array(1D array=w462, element=w458) -> (index of element=w459:i32)  [unwired: 1 in]
                n174 = Index Array(array=w461, index=w459) -> (element=w460:path)
                n175 = Greater Or Equal To 0?(x=w459) -> (x >= 0?=w457:bool)
              }
            }
          }
          n176 = case shown="\"Class\", Default" w415 {
            tunnel: w439 -> [_ w486]
            tunnel: w437 -> [w465 w485]
            tunnel: w432 -> [w463 w476]
            tunnel: [w472 w484] -> w429
            tunnel: w428 -> [w469 w483]
            tunnel: [w473 w482] -> w427
            tunnel: w420 -> [w466 w481]
            tunnel: w413 -> [w471 w480]
            tunnel: [w474 w479] -> w417
            tunnel: TRUE ("KeepLvClassRefOpen(False)") -> [w470 w478]
            tunnel: [TRUE FALSE] -> _
            tunnel: w410 -> [_ w475]
            frame "Interface" {
              n177 = Bundle By Name(cluster=T24 {"NewInterfaceFolder"=path "", "InterfaceName"="", "InterfaceDescription"="", "ParentInterfacesFilePath"=[], "FolderSuffix"="", "MethodsToCreate"=[]} ("CreateInterfaceType"), "InterfaceName"=w466, "InterfaceDescription"=w465, "ParentInterfacesFilePath"=w463) -> (w467:T24)
              n178 = call "GDSAPI_CreateInterface.vi"("KeepLvClassRefOpen(False)"=w470, "error in (no error)"=w471, "CreateInterfaceType"=w467, "ProjectItemToCreateClassUnder"=w469) -> ("error out"=w472:errorcluster, "LVClassLibraryRefnum"=w473:refnum<vi>, "LvClassFileOut"=w474:path)  [unwired: 5 in]
            }
            frame "Class", Default {
              n179 = Bundle By Name(cluster=T26 {"ClassProvider"=enum."GOOP-3(By reference)", "NewClassFolder"=path "", "ParentLvClassFilePath"=path "", "ClassName"="", "ClassDescription"="", "ClassTemplate"=enum."Standard", "ParentInterfacesFilePath"=[]} ("CreateClassType"), "ClassProvider"=w486, "ParentLvClassFilePath"=w475, "ClassName"=w481, "ClassDescription"=w485, "ParentInterfacesFilePath"=w476) -> (w487:T26)
              n180 = call "GDSAPI_CreateClass.vi"("KeepLvClassRefOpen(False)"=w478, "error in (no error)"=w480, "CreateClassType"=w487, "ProjectItemToCreateClassUnder"=w483) -> ("error out"=w484:errorcluster, "LVClassLibraryRefnum"=w482:refnum<vi>, "LvClassFileOut"=w479:path)  [unwired: 5 in]
            }
          }
          n181 = Format Into String(format string=" : %s", initial string=w424, w420) -> (resulting string=w423:string)  [unwired: 1 in, 1 out]
          n182 = property class="Str"(reference=w422, "Value"=w423) -> ()  [unwired: 1 in, 2 out]
          n183 = case shown="\"Interface\"" w415 {
            tunnel: w412 -> [w495 w504]
            tunnel: [w495 w503] -> w436
            tunnel: w420 -> [w489 w502]
            tunnel: [w496 w501] -> w435
            tunnel: w411 -> [w496 w500]
            tunnel: w417 -> [w490 w499]
            tunnel: w430 -> [w494 w498]
            tunnel: [w492 w498] -> w433
            tunnel: [w491 w497] -> w434
            tunnel: w431 -> [w493 w497]
            frame "Interface" {
              n184 = Build Array (concatenate)(w494, w489) -> (w492:string[])
              n185 = Build Array (concatenate)(w493, w490) -> (w491:path[])
            }
            frame "Class", Default {
              n186 = Build Array (concatenate)(w504, w502) -> (w503:string[])
              n187 = Build Array (concatenate)(w500, w499) -> (w501:path[])
            }
          }
          n188 = Bundle(cluster=T20 {"ClassNamn"="", "ClassPath"=path "", "InterfaceClass"=FALSE} ("Cluster"), "ClassNamn"=w420, "ClassPath"=w417, "InterfaceClass"=FALSE) -> (w426:T20)
          n189 = Build Array (concatenate)(w418, w426) -> (w419:T20[])
        }
        n190 = Bundle By Name(cluster=w407, "ClassPath"=w398, "ClassRefs"=w397, "ClassInfo"=w396) -> (w399:T21)
      }
      frame "CreateEnums" {
        n191 = Unbundle By Name(w516) -> ("ClassRefs"=w513:refnum<vi>[], "ClassPath"=w514:path[], "Classes"=w515:T11[], "ClassInfo"=w512:T20[])
        n192 = property class="Str"(reference=w507) -> (reference out=w506:refnum<vi>, "Value"=w505:string)  [unwired: 1 in, 1 out]
        n193 = for {
          tunnel: w515 -> [w528] mode=indexing
          tunnel: w514 -> [w526] mode=indexing
          tunnel: w513 -> [w525] mode=indexing
          shift-right: [w523] -> w508
          shift-left: w509 -> [w524]
          shift-right: [w521] -> w510
          shift-left: w512 -> [w522]
          tunnel: w506 -> [w520]
          tunnel: w505 -> [w519]
          n194 = Unbundle By Name(w528) -> ("Enums"=w527:T6[], "ClassName"=w518:string)
          n195 = for {
            tunnel: w527 -> [w553] mode=indexing
            tunnel: w526 -> [w540]
            tunnel: w525 -> [_]
            shift-right: [w551] -> w523
            shift-left: w524 -> [w552]
            shift-right: [w541] -> w521
            shift-left: w522 -> [w543]
            tunnel: w520 -> [w533]
            tunnel: w519 -> [w532]
            tunnel: w518 -> [w531]
            n196 = Unbundle By Name(w553) -> ("Name"=w530:string, "Items"=w547:string[], "Documentation"=w548:string)  [unwired: 4 out]
            n197 = Strip Path(path=w540) -> (stripped path=w538:path)  [unwired: 1 out]
            n198 = for {
              tunnel: w547 -> [w555] mode=indexing
              tunnel: T4 {"Name"="", "DataType"=enum."UINT8", "ArrayDim"=0, "CtrlPath"=path "", "DataTypeString"="", "AccessScope"=enum."public", "InitialData"=variant} -> [w556]
              tunnel: [w554] -> w545 mode=indexing
              n199 = Bundle By Name(cluster=w556, "Name"=w555) -> (w554:T4)
            }
            n200 = Concatenate Strings(w530, ".ctl" ("string")) -> (w537:string)
            n201 = Build Path(base path=w538, name or relative path=w537) -> (appended path=w536:path)
            n202 = call "Common_UpdateAttributes.vi"("ClassPath/LvClassRef"=w536, "NewAttributes"=w530, "ClassInfo"=w543, "error in (no error)"=w552, "Don't Prompt (False)"=TRUE, "Attributes"=w545, "Stereotype"="ENUM" ("regular expression"), "Ctl-Description"=w548) -> ("CtlPath"=w544:path, "error out"=w551:errorcluster)  [unwired: 9 in, 1 out]
            n203 = Format Into String(format string=" : %s", initial string=w532, w531) -> (resulting string=w535:string)  [unwired: 1 in, 1 out]
            n204 = Bundle(cluster=T20 {"ClassNamn"="", "ClassPath"=path "", "InterfaceClass"=FALSE} ("Cluster"), "ClassNamn"=w530, "ClassPath"=w544) -> (w542:T20)  [unwired: 1 in]
            n205 = property class="Str"(reference=w533, "Value"=w535) -> ()  [unwired: 1 in, 2 out]
            n206 = Build Array (concatenate)(w543, w542) -> (w541:T20[])
          }
        }
        n207 = Bundle By Name(cluster=w516, "ClassInfo"=w510) -> (w511:T21)
      }
      frame "CreateOusideStructs" {
        n208 = Unbundle By Name(w568) -> ("ClassInfo"=w567:T20[])  [unwired: 3 out]
        n209 = property class="Str"(reference=w562) -> (reference out=w561:refnum<vi>, "Value"=w560:string)  [unwired: 1 in, 1 out]
        n210 = for {
          shift-right: [w588] -> w563
          shift-left: w564 -> [w589]
          shift-right: [w581] -> w565
          shift-left: w567 -> [w583]
          tunnel: w561 -> [w574]
          tunnel: w560 -> [w573]
          tunnel: w558 -> [w572] mode=indexing
          tunnel: w557 -> [w571]
          n211 = Unbundle By Name(w572) -> ("Name"=w570:string, "Items"=w580:T4[], "Documentation"=w585:string)  [unwired: 2 out]
          n212 = Concatenate Strings(w570, ".ctl" ("string")) -> (w578:string)
          n213 = Build Path(base path=w571, name or relative path=w578) -> (appended path=w577:path)
          n214 = Format Into String(format string=" : %s", initial string=w573, w570) -> (resulting string=w576:string)  [unwired: 1 in, 1 out]
          n215 = property class="Str"(reference=w574, "Value"=w576) -> ()  [unwired: 1 in, 2 out]
          n216 = call "Common_UpdateAttributes.vi"("ClassPath/LvClassRef"=w577, "NewAttributes"=w570, "ClassInfo"=w583, "error in (no error)"=w589, "Don't Prompt (False)"=TRUE, "Attributes"=w580, "Stereotype"="STRUCT" ("regular expression"), "Ctl-Description"=w585) -> ("CtlPath"=w584:path, "error out"=w588:errorcluster)  [unwired: 9 in, 1 out]
          n217 = Bundle(cluster=T20 {"ClassNamn"="", "ClassPath"=path "", "InterfaceClass"=FALSE} ("Cluster"), "ClassNamn"=w570, "ClassPath"=w584) -> (w582:T20)  [unwired: 1 in]
          n218 = Build Array (concatenate)(w583, w582) -> (w581:T20[])
        }
        n219 = Bundle By Name(cluster=w568, "ClassInfo"=w565) -> (w566:T21)
      }
      frame "CreateStruct" {
        n220 = Unbundle By Name(w602) -> ("ClassRefs"=w599:refnum<vi>[], "ClassPath"=w600:path[], "Classes"=w601:T11[], "ClassInfo"=w598:T20[])
        n221 = property class="Str"(reference=w592) -> (reference out=w591:refnum<vi>, "Value"=w590:string)  [unwired: 1 in, 1 out]
        n222 = for {
          tunnel: w601 -> [w613] mode=indexing
          tunnel: w600 -> [w611] mode=indexing
          tunnel: w599 -> [w610] mode=indexing
          shift-right: [w608] -> w594
          shift-left: w595 -> [w609]
          shift-right: [w606] -> w596
          shift-left: w598 -> [w607]
          tunnel: w591 -> [w605]
          tunnel: w590 -> [w604]
          n223 = Unbundle By Name(w613) -> ("Structs"=w612:T1[], "ClassName"=w603:string)
          n224 = for {
            tunnel: w612 -> [w636] mode=indexing
            tunnel: w611 -> [w622]
            tunnel: w610 -> [_]
            shift-right: [w634] -> w608
            shift-left: w609 -> [w635]
            shift-right: [w627] -> w606
            shift-left: w607 -> [w629]
            tunnel: w605 -> [w618]
            tunnel: w604 -> [w617]
            tunnel: w603 -> [w615]
            n225 = Unbundle By Name(w636) -> ("Name"=w616:string, "Items"=w626:T4[], "Documentation"=w631:string)  [unwired: 2 out]
            n226 = Strip Path(path=w622) -> (stripped path=w624:path)  [unwired: 1 out]
            n227 = Concatenate Strings(w616, ".ctl" ("string")) -> (w623:string)
            n228 = Build Path(base path=w624, name or relative path=w623) -> (appended path=w621:path)
            n229 = Format Into String(format string=" : %s", initial string=w617, w615) -> (resulting string=w620:string)  [unwired: 1 in, 1 out]
            n230 = property class="Str"(reference=w618, "Value"=w620) -> ()  [unwired: 1 in, 2 out]
            n231 = call "Common_UpdateAttributes.vi"("ClassPath/LvClassRef"=w621, "NewAttributes"=w616, "ClassInfo"=w629, "error in (no error)"=w635, "Don't Prompt (False)"=TRUE, "Attributes"=w626, "Stereotype"="STRUCT" ("regular expression"), "Ctl-Description"=w631) -> ("CtlPath"=w630:path, "error out"=w634:errorcluster)  [unwired: 9 in, 1 out]
            n232 = Bundle(cluster=T20 {"ClassNamn"="", "ClassPath"=path "", "InterfaceClass"=FALSE} ("Cluster"), "ClassNamn"=w616, "ClassPath"=w630) -> (w628:T20)  [unwired: 1 in]
            n233 = Build Array (concatenate)(w629, w628) -> (w627:T20[])
          }
        }
        n234 = Bundle By Name(cluster=w602, "ClassInfo"=w596) -> (w597:T21)
      }
      frame "UpdateAttribute" {
        n235 = Unbundle By Name(w645) -> ("ClassRefs"=w646:refnum<vi>[], "ClassPath"=w647:path[], "Classes"=w648:T11[], "ClassInfo"=w642:T20[])
        n236 = property class="Str"(reference=w641) -> (reference out=w640:refnum<vi>, "Value"=w639:string)  [unwired: 1 in, 1 out]
        n237 = for {
          tunnel: w648 -> [w654] mode=indexing
          tunnel: w647 -> [_] mode=indexing
          tunnel: w646 -> [w664] mode=indexing
          shift-right: [w662] -> w643
          shift-left: w644 -> [w663]
          tunnel: w642 -> [w661]
          tunnel: w640 -> [w657]
          tunnel: w639 -> [w655]
          tunnel: [w650] -> w637 mode=indexing
          n238 = Unbundle By Name(w654) -> ("Attributes"=w653:T4[])
          n239 = Unbundle By Name(w654) -> ("Methods"=w652:T12[], "ClassName"=w656:string)
          n240 = Format Into String(format string=" : %s", initial string=w655, w656) -> (resulting string=w659:string)  [unwired: 1 in, 1 out]
          n241 = call "Common_UpdateAttributes.vi"("ClassPath/LvClassRef"=w664, "ClassInfo"=w661, "error in (no error)"=w663, "Don't Prompt (False)"=TRUE, "Attributes"=w653) -> ("error out"=w662:errorcluster)  [unwired: 12 in, 2 out]
          n242 = property class="Str"(reference=w657, "Value"=w659) -> ()  [unwired: 1 in, 2 out]
          n243 = for {
            tunnel: w653 -> [w669] mode=indexing
            shift-right: [w665] -> w651
            shift-left: w652 -> [w666]
            n244 = Unbundle By Name(w669) -> ("AccessScope"=w668:T2, "Name"=w667:string)
            n245 = case shown="\"public\"" w668 {
              tunnel: w667 -> [w672 _]
              tunnel: w666 -> [w674 w688]
              tunnel: [w680 w688] -> w665
              frame "public" {
                w676 = TRUE
                n246 = for {
                  tunnel: w674 -> [w687] mode=indexing
                  tunnel: [w686] -> w673 mode=indexing
                  n247 = Unbundle By Name(w687) -> ("MethodName"=w686:string)
                }
                n248 = Search 1D Array(1D array=w673, element=w672) -> (index of element=w671:i32)  [unwired: 1 in]
                n249 = Greater Or Equal To 0?(x=w671) -> (x >= 0?=w670:bool)
                n250 = Format Into String(format string="Attribute %s is public, therefor accessory methods have been created." ("regular expression"), w672) -> (resulting string=w678:string)  [unwired: 2 in, 1 out]
                n251 = Bundle By Name(cluster=T12 {"ReturnType"={"Name"="", "DataType"=enum."UINT8", "ArrayDim"=0, "CtrlPath"=path "", "DataTypeString"="", "AccessScope"=enum."public", "InitialData"=variant}, "MethodName"="", "AccessScope"=enum."public", "Modifiers"=[], "MethodDocumentation"="", "MethodContent"="", "MethodArguments"=[], "GetProperty"={"Active"=FALSE, "AccessScope"=enum."public", "Code"=""}, "SetProperty"={"Active"=FALSE, "AccessScope"=enum."public", "Code"=""}}, "MethodName"=w672, "AccessScope"=GDSString_AccessScopeModifierType."public", "MethodDocumentation"=w678, "GetProperty.Active"=w676, "SetProperty.Active"=w676) -> (w681:T12)
                n252 = case shown="False" w670 {
                  tunnel: w681 -> [w684 _]
                  tunnel: [w683 w685] -> w680
                  tunnel: w674 -> [w682 w685]
                  frame False {
                    n253 = Build Array (concatenate)(w684, w682) -> (w683:T12[])
                  }
                  frame True {
                  }
                }
              }
              frame Default {
              }
            }
          }
          n254 = Bundle By Name(cluster=w654, "Methods"=w651) -> (w650:T11)
        }
        n255 = Bundle By Name(cluster=w645, "Classes"=w637) -> (w638:T21)
      }
      frame "UpdateParentClassTypes" {
        n256 = Unbundle By Name(w690) -> ("ClassPath"=w697:path[], "Classes"=w689:T11[])
        n257 = for {
          tunnel: [w700] -> w696 mode=indexing
          tunnel: [w699] -> w695 mode=indexing
          tunnel: w689 -> [w698] mode=indexing
          n258 = Unbundle By Name(w698) -> ("ClassName"=w700:string, "ClassType"=w699:T15)
        }
        n259 = for {
          tunnel: w697 -> [_] mode=indexing
          tunnel: w689 -> [w703] mode=indexing
          tunnel: w696 -> [w706]
          tunnel: w695 -> [w705]
          tunnel: [w701] -> w693 mode=indexing
          n260 = Unbundle By Name(w703) -> ("ParentClasses"=w704:T14[])  [unwired: 1 out]
          n261 = Unbundle By Name(w703) -> ()  [unwired: 1 out]
          n262 = for {
            tunnel: w704 -> [w714] mode=indexing
            tunnel: w706 -> [w712]
            tunnel: w705 -> [w709]
            tunnel: [w713] -> w702 mode=indexing
            n263 = Unbundle By Name(w714) -> ("ClassName"=w711:string, "ClassType"=w707:T15)
            n264 = Search 1D Array(1D array=w712, element=w711) -> (index of element=w710:i32)  [unwired: 1 in]
            n265 = case shown="-1" w710 {
              selector: w710 -> [w716 _]
              tunnel: w709 -> [w717 _]
              tunnel: [w715 w718] -> w708
              tunnel: w707 -> [_ w720]
              frame 0, Default {
                n266 = Index Array(array=w717, index=w716) -> (element=w715:T15)
              }
              frame -1 {
                n267 = Equal?(x=w720, y=GDSString_ClassType."Undefined") -> (x = y?=w721:bool)
                n268 = Select(t=GDSString_ClassType."Class" ("y"), s=w721, f=w720) -> (s? t:f=w718:T15)
              }
            }
            n269 = Bundle By Name(cluster=w714, "ClassType"=w708) -> (w713:T14)
          }
          n270 = Bundle By Name(cluster=w703, "ParentClasses"=w702) -> (w701:T11)
        }
        n271 = Bundle By Name(cluster=w690, "Classes"=w693) -> (w692:T21)
      }
      frame "UpdateMethodTypes" {
        n272 = Unbundle By Name(w724) -> ("ClassPath"=w730:path[], "Classes"=w729:T11[], "ClassInfo"=w723:T20[])
        n273 = for {
          tunnel: w730 -> [_] mode=indexing
          tunnel: w729 -> [w733] mode=indexing
          tunnel: w723 -> [w735]
          tunnel: [w731] -> w727 mode=indexing
          n274 = Unbundle By Name(w733) -> ("Methods"=w734:T12[])  [unwired: 1 out]
          n275 = Unbundle By Name(w733) -> ()  [unwired: 1 out]
          n276 = for {
            tunnel: w734 -> [w742] mode=indexing
            tunnel: w735 -> [w743]
            tunnel: [w740] -> w732 mode=indexing
            n277 = Unbundle By Name(w742) -> ("ReturnType"=w737:T4, "MethodArguments"=w744:T4[])
            n278 = for {
              tunnel: w744 -> [w754] mode=indexing
              tunnel: w743 -> [w753]
              tunnel: [w752] -> w741 mode=indexing
              n279 = call "CommonVIs_UpdateAttributeCtrlPath.vi"("ClassInfo"=w753, "DataType in"=w754) -> ("DataType out"=w752:T4)  [unwired: 9 in]
            }
            n280 = Unbundle By Name(w737) -> ("Name"=w736:string)
            n281 = call "CommonVIs_UpdateAttributeCtrlPath.vi"("ClassInfo"=w743, "DataType in"=w737) -> ("DataType out"=w738:T4)  [unwired: 9 in]
            n282 = case shown="\"\"" w736 {
              selector: w736 -> [_ w749]
              tunnel: [w745 w751] -> w739
              tunnel: w738 -> [w745 w750]
              frame Default {
              }
              frame "" {
                n283 = Unbundle By Name(w750) -> ("DataType"=w747:T5)
                n284 = Format Into String(format string="%s Return(%s)", w749, w747) -> (resulting string=w746:string)  [unwired: 2 in, 1 out]
                n285 = Bundle By Name(cluster=w750, "Name"=w746) -> (w751:T4)
              }
            }
            n286 = Bundle By Name(cluster=w742, "ReturnType"=w739, "MethodArguments"=w741) -> (w740:T12)
          }
          n287 = Bundle By Name(cluster=w733, "Methods"=w732) -> (w731:T11)
        }
        n288 = Bundle By Name(cluster=w724, "Classes"=w727) -> (w726:T21)
      }
      frame "UpdateConstructors" {
        n289 = Unbundle By Name(w759) -> ("ClassPath"=w763:path[], "Classes"=w762:T11[], "ClassRefs"=w757:refnum<vi>[])
        n290 = for {
          tunnel: w763 -> [_] mode=indexing
          tunnel: w762 -> [w777] mode=indexing
          tunnel: [w775] -> w761 mode=indexing
          tunnel: w757 -> [w774] mode=indexing
          shift-right: [w764] -> w755
          shift-left: w756 -> [w772]
          n291 = Unbundle By Name(w777) -> ("ClassName"=w771:string, "Methods"=w778:T12[])
          n292 = call "GDSLvClass_GetClassMethod.vi"("Class Refnum In"=w774, "VINames"=string[] ["Create", "Init"], "error in (no error)"=w772) -> ("ViPaths"=w768:path[], "error out"=w764:errorcluster)  [unwired: 13 in, 2 out]
          n293 = for {
            tunnel: w778 -> [w807] mode=indexing
            tunnel: [w807] -> w776 mode=indexing if=w805
            tunnel: w771 -> [w808]
            tunnel: [w807] -> w770 mode=indexing if=w806
            n294 = Unbundle By Name(w807) -> ("MethodName"=w809:string)
            n295 = Equal?(x=w808, y=w809) -> (x = y?=w806:bool)
            n296 = Not(x=w806) -> (.not. x?=w805:bool)
          }
          n297 = for {
            tunnel: w768 -> [w779] mode=indexing
            tunnel: [w780] -> w766
            tunnel: [w779] -> w765
            stop <- w780 continue-if-true
            n298 = Empty String/Path?(string/path=w779) -> (empty?=w780:bool)
          }
          n299 = Empty Array?(array=w770) -> (empty?=w769:bool)
          n300 = Or(x=w769, y=w766) -> (x .or. y?=w767:bool)
          n301 = case shown="False" w767 {
            tunnel: w777 -> [w799 w804]
            tunnel: w776 -> [w798 _]
            tunnel: [w797 w804] -> w775
            tunnel: w770 -> [w795 _]
            tunnel: w765 -> [w782 _]
            frame False {
              w787 = "%s" ("format string")
              w788 = "\n\n" ("delimiter (Tab)")
              n302 = for {
                tunnel: w795 -> [w803] mode=indexing
                tunnel: [w803] -> w796
                tunnel: [w802] -> w792 mode=concatenating
                tunnel: [w801] -> w791 mode=indexing
                tunnel: [w800] -> w789 mode=indexing
                n303 = Unbundle By Name(w803) -> ("MethodArguments"=w802:T4[], "MethodDocumentation"=w801:string, "MethodContent"=w800:string)
              }
              n304 = call <vilib>:"Get File Extension.vi"("file"=w782) -> ("filename without extension"=w781:string)  [unwired: 6 in, 4 out]
              n305 = Array To Spreadsheet String(delimiter (Tab)=w788, array=w791, 3:w787) -> (spreadsheet string=w790:string)
              n306 = Array To Spreadsheet String(delimiter (Tab)=w788, array=w789, 3:w787) -> (spreadsheet string=w786:string)
              n307 = call <vilib>:"Trim Whitespace.vi"("string"=w790) -> ("trimmed string"=w785:string)  [unwired: 1 in]
              n308 = call <vilib>:"Trim Whitespace.vi"("string"=w786) -> ("trimmed string"=w784:string)  [unwired: 1 in]
              n309 = Bundle By Name(cluster=w796, "ReturnType"=T4 {"Name"="", "DataType"=enum."void", "ArrayDim"=0, "CtrlPath"=path "", "DataTypeString"="", "AccessScope"=enum."public", "InitialData"=variant}, "MethodArguments"=w792, "MethodDocumentation"=w785, "MethodContent"=w784, "MethodName"=w781) -> (w783:T12)
              n310 = Build Array (concatenate)(w798, w783) -> (w794:T12[])
              n311 = Bundle By Name(cluster=w799, "Methods"=w794) -> (w797:T11)
            }
            frame True {
            }
          }
        }
        n312 = Bundle By Name(cluster=w759, "Classes"=w761) -> (w760:T21)
      }
      frame "UpdateDestructors" {
        n313 = Unbundle By Name(w814) -> ("ClassPath"=w818:path[], "Classes"=w817:T11[], "ClassRefs"=w812:refnum<vi>[])
        n314 = for {
          tunnel: w818 -> [_] mode=indexing
          tunnel: w817 -> [w832] mode=indexing
          tunnel: [w830] -> w816 mode=indexing
          tunnel: w812 -> [w829] mode=indexing
          shift-right: [w819] -> w810
          shift-left: w811 -> [w827]
          n315 = Unbundle By Name(w832) -> ("ClassName"=w826:string, "Methods"=w833:T12[])
          n316 = for {
            tunnel: w833 -> [w869] mode=indexing
            tunnel: [w869] -> w831 mode=indexing if=w868
            tunnel: w826 -> [w867]
            tunnel: [w869] -> w825 mode=indexing if=w862
            n317 = Unbundle By Name(w869) -> ("MethodName"=w865:string)
            n318 = Format Into String(format string="~%s", w867) -> (resulting string=w866:string)  [unwired: 2 in, 1 out]
            n319 = Equal?(x="finalize", y=w865) -> (x = y?=w864:bool)
            n320 = Equal?(x=w866, y=w865) -> (x = y?=w863:bool)
            n321 = Or(x=w864, y=w863) -> (x .or. y?=w862:bool)
            n322 = Not(x=w862) -> (.not. x?=w868:bool)
          }
          n323 = call "GDSLvClass_GetClassMethod.vi"("Class Refnum In"=w829, "VINames"=string[] ["Destroy", "CleanUp"], "error in (no error)"=w827) -> ("ViPaths"=w823:path[], "error out"=w819:errorcluster)  [unwired: 13 in, 2 out]
          n324 = for {
            tunnel: w823 -> [w834] mode=indexing
            tunnel: [w835] -> w821
            tunnel: [w834] -> w820
            stop <- w835 continue-if-true
            n325 = Empty String/Path?(string/path=w834) -> (empty?=w835:bool)
          }
          n326 = Empty Array?(array=w825) -> (empty?=w824:bool)
          n327 = Or(x=w824, y=w821) -> (x .or. y?=w822:bool)
          n328 = case shown="False" w822 {
            tunnel: w832 -> [w854 w859]
            tunnel: w831 -> [w853 _]
            tunnel: [w852 w859] -> w830
            tunnel: w825 -> [w850 _]
            tunnel: w820 -> [w837 _]
            frame False {
              w842 = "%s" ("format string")
              w843 = "\n\n" ("delimiter (Tab)")
              n329 = for {
                tunnel: w850 -> [w858] mode=indexing
                tunnel: [w858] -> w851
                tunnel: [w857] -> w847 mode=concatenating
                tunnel: [w856] -> w846 mode=indexing
                tunnel: [w855] -> w844 mode=indexing
                n330 = Unbundle By Name(w858) -> ("MethodArguments"=w857:T4[], "MethodDocumentation"=w856:string, "MethodContent"=w855:string)
              }
              n331 = call <vilib>:"Get File Extension.vi"("file"=w837) -> ("filename without extension"=w836:string)  [unwired: 6 in, 4 out]
              n332 = Array To Spreadsheet String(delimiter (Tab)=w843, array=w846, 3:w842) -> (spreadsheet string=w845:string)
              n333 = Array To Spreadsheet String(delimiter (Tab)=w843, array=w844, 3:w842) -> (spreadsheet string=w841:string)
              n334 = call <vilib>:"Trim Whitespace.vi"("string"=w845) -> ("trimmed string"=w840:string)  [unwired: 1 in]
              n335 = call <vilib>:"Trim Whitespace.vi"("string"=w841) -> ("trimmed string"=w839:string)  [unwired: 1 in]
              n336 = Bundle By Name(cluster=w851, "ReturnType"=T4 {"Name"="", "DataType"=enum."void", "ArrayDim"=0, "CtrlPath"=path "", "DataTypeString"="", "AccessScope"=enum."public", "InitialData"=variant}, "MethodArguments"=w847, "MethodDocumentation"=w840, "MethodContent"=w839, "MethodName"=w836) -> (w838:T12)
              n337 = Build Array (concatenate)(w853, w838) -> (w849:T12[])
              n338 = Bundle By Name(cluster=w854, "Methods"=w849) -> (w852:T11)
            }
            frame True {
            }
          }
        }
        n339 = Bundle By Name(cluster=w814, "Classes"=w816) -> (w815:T21)
      }
      frame "AddInterfaceMethods" {
        n340 = property class="Str"(reference=w873) -> (reference out=w872:refnum<vi>, "Value"=w871:string)  [unwired: 1 in, 1 out]
        n341 = Unbundle By Name(w874) -> ("ClassPath"=w878:path[], "Classes"=w877:T11[])  [unwired: 1 out]
        n342 = for {
          shift-right: [w888] -> w875
          shift-left: w876 -> [w889]
          tunnel: w878 -> [w880] mode=indexing
          tunnel: w877 -> [w881] mode=indexing
          tunnel: w872 -> [w884]
          tunnel: w871 -> [w883]
          n343 = Unbundle By Name(w881) -> ("Methods"=w887:T12[], "ClassName"=w882:string)
          n344 = Unbundle By Name(w881) -> ("ClassType"=w879:T15)
          n345 = case shown="\"Interface\"" w879 {
            tunnel: w889 -> [w890 w894]
            tunnel: [w890 w893] -> w888
            tunnel: w887 -> [_ w891]
            tunnel: w880 -> [_ w892]
            frame Default {
            }
            frame "Interface" {
              n346 = call "GDSAPI_CreateMethods2.vi"("error in (no error)"=w894, "Methods"=w891, "ClassPath(*.lvclass)"=w892) -> ("error out"=w893:errorcluster)  [unwired: 7 in, 1 out]
            }
          }
          n347 = Format Into String(format string=" : %s", initial string=w883, w882) -> (resulting string=w886:string)  [unwired: 1 in, 1 out]
          n348 = property class="Str"(reference=w884, "Value"=w886) -> ()  [unwired: 1 in, 2 out]
        }
      }
      frame "CreateMethods" {
        n349 = property class="Str"(reference=w898) -> (reference out=w897:refnum<vi>, "Value"=w896:string)  [unwired: 1 in, 1 out]
        n350 = Unbundle By Name(w899) -> ("ClassPath"=w903:path[], "Classes"=w902:T11[])
        n351 = for {
          shift-right: [w914] -> w900
          shift-left: w901 -> [w916]
          tunnel: w903 -> [w915] mode=indexing
          tunnel: w902 -> [w907] mode=indexing
          tunnel: w897 -> [w910]
          tunnel: w896 -> [w909]
          tunnel: w895 -> [w905]
          n352 = Unbundle By Name(w907) -> ("Methods"=w913:T12[], "ClassName"=w908:string)
          n353 = Unbundle By Name(w907) -> ("ClassType"=w906:T15)
          n354 = case shown="\"Class\", Default" w906 {
            tunnel: w916 -> [w917 w922]
            tunnel: w915 -> [_ w921]
            tunnel: [w917 w920] -> w914
            tunnel: w913 -> [_ w919]
            tunnel: w905 -> [_ w918]
            frame "Interface" {
            }
            frame "Class", Default {
              n355 = call "GDSAPI_CreateMethods2.vi"("PropertyMethodType"=w918, "error in (no error)"=w922, "Methods"=w919, "ClassPath(*.lvclass)"=w921) -> ("error out"=w920:errorcluster)  [unwired: 6 in, 1 out]
            }
          }
          n356 = Format Into String(format string=" : %s", initial string=w909, w908) -> (resulting string=w912:string)  [unwired: 1 in, 1 out]
          n357 = property class="Str"(reference=w910, "Value"=w912) -> ()  [unwired: 1 in, 2 out]
        }
      }
      frame "AddExtraClasses?" {
        n358 = Unbundle By Name(w924) -> ("Proj"=w923:refnum<vi>)
        n359 = for {
          tunnel: w927 -> [w939]
          tunnel: T28 [{"ClassName"="Console_class.zip", "SearchPattern"=["System.out.print", "Console.Write"]}] -> [w938] mode=indexing
          tunnel: w925 -> [w932]
          tunnel: w923 -> [w931]
          n360 = Unbundle By Name(w938) -> ("ClassName"=w934:string, "SearchPattern"=w937:string[])
          n361 = for {
            tunnel: w939 -> [w954] mode=indexing
            tunnel: w937 -> [w952]
            tunnel: [w951] -> w930
            stop <- w951 stop-if-true
            n362 = Unbundle By Name(w954) -> ("Methods"=w953:T12[])
            n363 = for {
              tunnel: w953 -> [w958] mode=indexing
              tunnel: w952 -> [w956]
              tunnel: [w955] -> w951
              stop <- w955 stop-if-true
              n364 = Unbundle By Name(w958) -> ("MethodContent"=w957:string)
              n365 = for {
                tunnel: w957 -> [w962]
                tunnel: w956 -> [w961] mode=indexing
                tunnel: [w959] -> w955
                stop <- w959 stop-if-true
                n366 = Match Pattern(string=w962, regular expression=w961) -> (offset past match=w960:i32)  [unwired: 1 in, 3 out]
                n367 = Greater Or Equal To 0?(x=w960) -> (x >= 0?=w959:bool)
              }
            }
          }
          n368 = Current VI's Path() -> (path=w936:path)
          n369 = Strip Path(path=w936) -> (stripped path=w935:path)  [unwired: 1 out]
          n370 = Build Path(base path=w935, name or relative path=w934) -> (appended path=w933:path)
          n371 = case shown="True" w930 {
            tunnel: w933 -> [_ w945]
            tunnel: w932 -> [_ w944]
            tunnel: w931 -> [_ w942]
            frame False {
            }
            frame True {
              n372 = call <vilib>:"Unzip.vi"("Target directory (same as Zip file if empty)"=w944, "Zip file"=w945) -> ("Unzipped files"=w943:path[])  [unwired: 7 in, 2 out]
              n373 = for {
                tunnel: w943 -> [w950] mode=indexing
                tunnel: [w946] -> w940
                stop <- w947 stop-if-true
                n374 = call <vilib>:"Get File Extension.vi"("file"=w950) -> ("lowercase file extension"=w949:string, "dup file"=w946:path)  [unwired: 6 in, 3 out]
                n375 = Equal?(x=w949, y="lvclass") -> (x = y?=w947:bool)
              }
              n376 = property class="Project"(reference=w942) -> ("My Computer"=w941:refnum<vi>)  [unwired: 1 in, 2 out]
              n377 = invoke class="TargetItem" method="AddFile"(reference=w941, "Path"=w940) -> ()  [unwired: 2 in, 4 out]
            }
          }
        }
      }
      frame "SaveAll" {
        w968 = TRUE ("ExcludeDependencies")
        n378 = Unbundle By Name(w971) -> ("Proj"=w970:refnum<vi>)  [unwired: 3 out]
        n379 = property class="Project"(reference=w970) -> ("My Computer"=w969:refnum<vi>)  [unwired: 1 in, 2 out]
        n380 = invoke class="TargetItem" method="Get All Descendents"(reference=w969, "Exclude Dependencies"=w968, "ExcludeBuilds"=w968, "ExcludeTargets"=w968) -> (reference out=w963:refnum<vi>, "All Descendents"=w965:refnum<vi>[])  [unwired: 3 in, 5 out]
        n381 = for {
          tunnel: w965 -> [w977] mode=indexing
          tunnel: [w973] -> w966
          n382 = property class="ProjectItem"(reference=w977) -> (reference out=w974:refnum<vi>, error out=w973:errorcluster, "Reference"=w975:refnum<vi>)  [unwired: 1 in]
          n383 = Not A Number/Path/Refnum?(number/path/refnum=w975) -> (NaN/Path/Refnum?=w976:bool)
          n384 = case shown="True" w976 {
            tunnel: w975 -> [w980 _]
            tunnel: w974 -> [_ w984]
            frame False {
              n385 = invoke class="VI" method="Save.Instrument"(reference=w980) -> (reference out=w978:refnum<vi>, error out=w979:errorcluster)  [unwired: 5 in, 4 out]
              n386 = Close Reference(reference=w978, error in (no error)=w979) -> ()  [unwired: 1 out]
            }
            frame True {
              w983 = refnum<vi> refnum  # LVClassLibrary
              n387 = To More Specific Class(target class=w983, reference=w984) -> (specific class reference=w981:refnum<vi>, error out=w982:errorcluster)  [unwired: 1 in]
              n388 = case shown="No Error" w982 {
                tunnel: w981 -> [w985 _]
                frame No Error {
                  n389 = invoke class="LVClassLibrary" method="Save"(reference=w985) -> ()  [unwired: 3 in, 4 out]
                }
                frame Error {
                }
              }
            }
          }
        }
        n390 = Close Reference(reference=w965, error in (no error)=w966) -> (error out=w964:errorcluster)
        n391 = Close Reference(reference=w963, error in (no error)=w964) -> ()  [unwired: 1 out]
      }
      frame "Done" {
        n392 = Unbundle By Name(w1009) -> ("StartTime"=w998:timestamp, "App"=w1002:refnum<vi>, "Proj"=w1008:refnum<vi>, "ProjItem"=w1006:refnum<vi>)
        n393 = Close Reference(reference=w1006, error in (no error)=w1001) -> (error out=w1005:errorcluster)
        n394 = invoke class="Project" method="Save"(reference=w1008, error in=w1005) -> (reference out=w1004:refnum<vi>, error out=w1007:errorcluster)  [unwired: 2 in, 2 out]
        n395 = Close Reference(reference=w1004, error in (no error)=w1007) -> (error out=w1003:errorcluster)
        n396 = Close Reference(reference=w1002, error in (no error)=w1003) -> (error out=w1000:errorcluster)
        n397 = Get Date/Time In Seconds() -> (seconds since 1Jan1904=w999:timestamp)
        n398 = Subtract(x=w999, y=w998) -> (x-y=w997:dbl)
        n399 = Quotient & Remainder(x=w997, y=60.0) -> (x-y*floor(x/y)=w987:dbl, floor(x/y)=w988:dbl)
        n400 = property class="Str"(reference=w990) -> (reference out=w992:refnum<vi>, "Value"=w994:string)  [unwired: 1 in, 1 out]
        n401 = Format Into String(format string="Conversion completed in %d min %02d s", w988, w987) -> (resulting string=w986:string)  [unwired: 2 in, 1 out]
        n402 = Concatenate Strings(w994, "\n" ("string"), w986) -> (w993:string)
        n403 = property class="Str"(reference=w992, "Value"=w993, "Text.Scroll Position"=u32 4294967295) -> ()  [unwired: 1 in, 2 out]
      }
      frame "CloseDown", "Error", Default {
        n404 = call "CommonVIs_UmlOpenVIRef.vi"("ProjectNameIn"="clear", "error in"=w1012) -> ("error out"=w1011:errorcluster)  [unwired: 6 in, 3 out]
      }
    }
    n405 = Unbundle By Name(w35) -> ("Classes"=→"ClassesOut":T11[])
    n406 = Equal?(x=w54, y="Exit") -> (x = y?=w52:bool)
    n407 = Select(t="Error", s=w57, f=w54) -> (s? t:f=w55:string)
  }
  "error out" <- w20
  n408 = Unbundle By Name(w6) -> ("Pattern-Before"=w5:T10)
  n409 = call "GDSAPI_SetClassOptions.vi"("SetAction(Set All)"=GDSAPI_SetClassOptionsAction."Set Pattern Type", "PatternIn"=w5) -> ()  [unwired: 6 in, 4 out]
